vi "FixJKIHelper.vi"() -> ()   [LabVIEW 2017]
uses:
  _Support/Common/Format Timestamp.vi
  _Shared/CSM Shared.lvlib
  _csmDoc/csmdoc.lvlib
  Communicable State Machine.lvlib
  user32.dll
panel:
  out "String Cache":string
  in  "Bottom Right":string
  in  "Bottom Left":string
  out "2D Picture":picture
  in  "Error in":errorcluster caption="error in (no error)"
  out "Listbox":i32(listbox)
  in  "Progress Bar":u8(slide) scale=-1.0..292.0
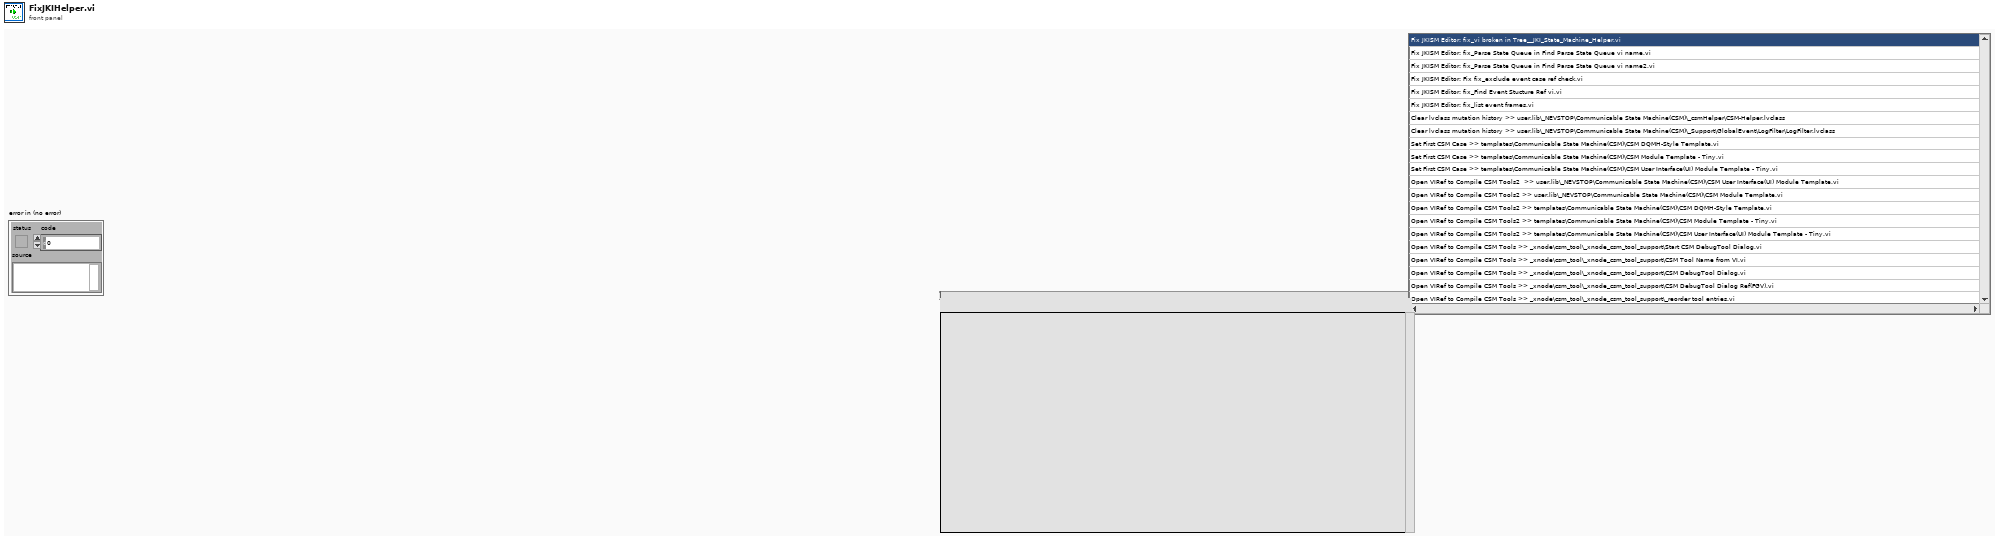
[diagram p1: front panel]
types:
  T1 = enum32{"Invalid", "Standard", "Closed", "Hidden", "Minimized", "Maximized"}
  T2 = enum32{"invalid app kind", "Development System", "Run Time System", "Student Edition", "Embedded LabVIEW", "Evaluation", "Custom"}
  T3 = cluster{"Core":cluster{"Current VI Reference":refnum<vi>, "Close Panel on Exit?":bool}, "Listbox Symbols":i32[], "Listbox Index":i32, "_JKI State Machine Helper VIs":path[], "CSM Templates":path[], "CSM lvclass":path[], "_JKI State Machine Helper Folders":path[], "Actions":string[], "LangID":string, "DescMap":variant, "NoteMap":variant, "Polish":cluster{"Version":refnum<vi>, "Action":refnum<vi>, "Progress Bar":refnum<vi>, "2D Picture":refnum<vi>, "Hold":bool, "Slides":picture[]}}
  T4 = cluster{"Version":refnum<vi>, "Action":refnum<vi>, "Progress Bar":refnum<vi>, "2D Picture":refnum<vi>, "Hold":bool, "Slides":picture[]}
  T5 = cluster{"Current VI Reference":refnum<vi>, "Close Panel on Exit?":bool}
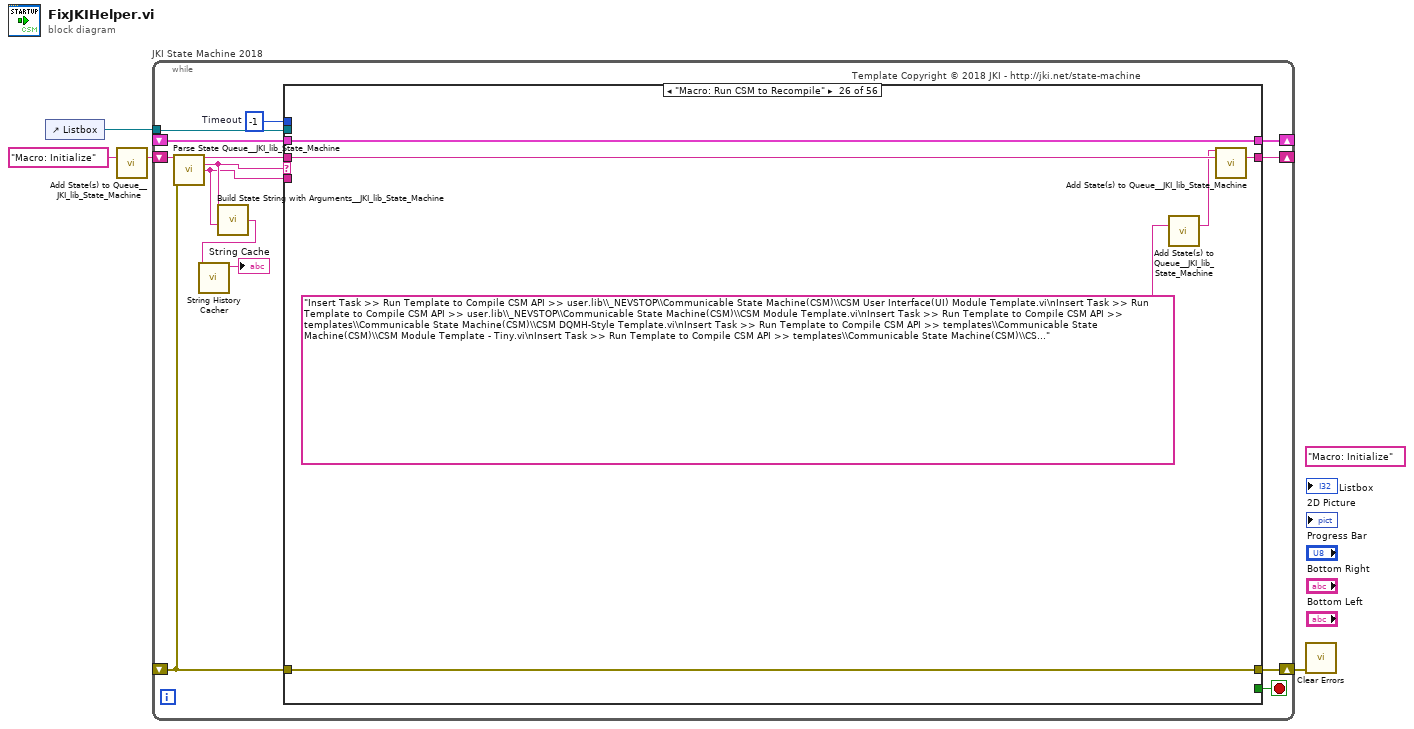
[diagram p0: block diagram]
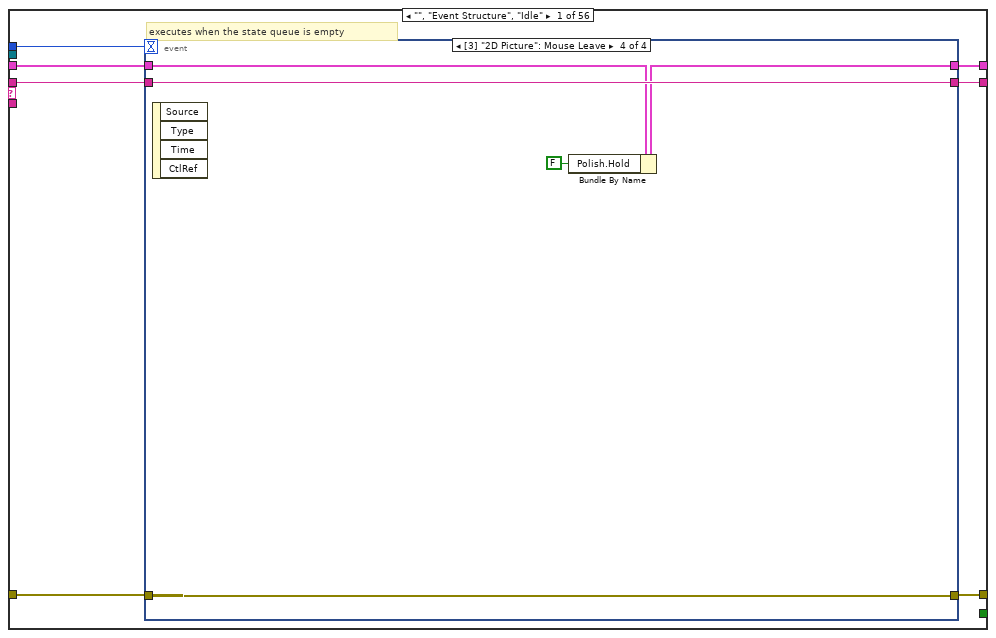
[diagram p2: hidden frame]
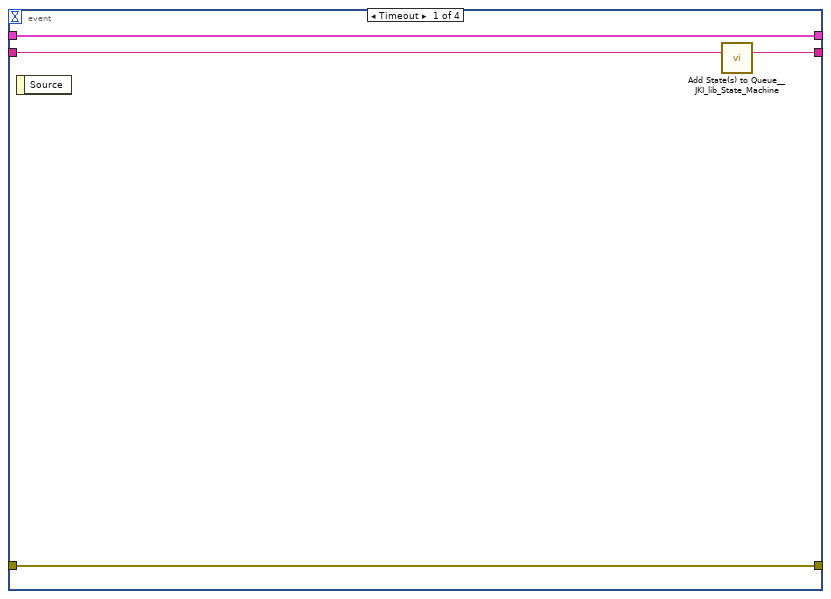
[diagram p3: hidden frame]
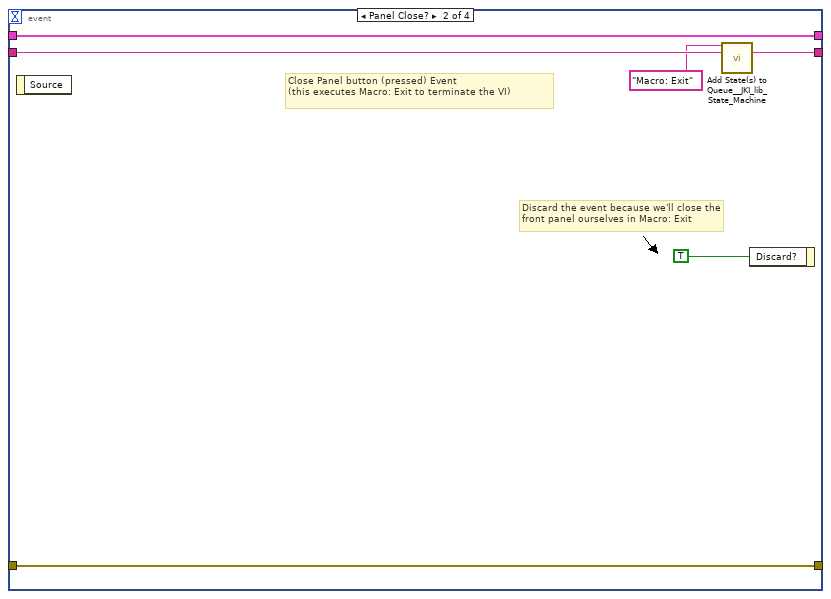
[diagram p4: hidden frame]
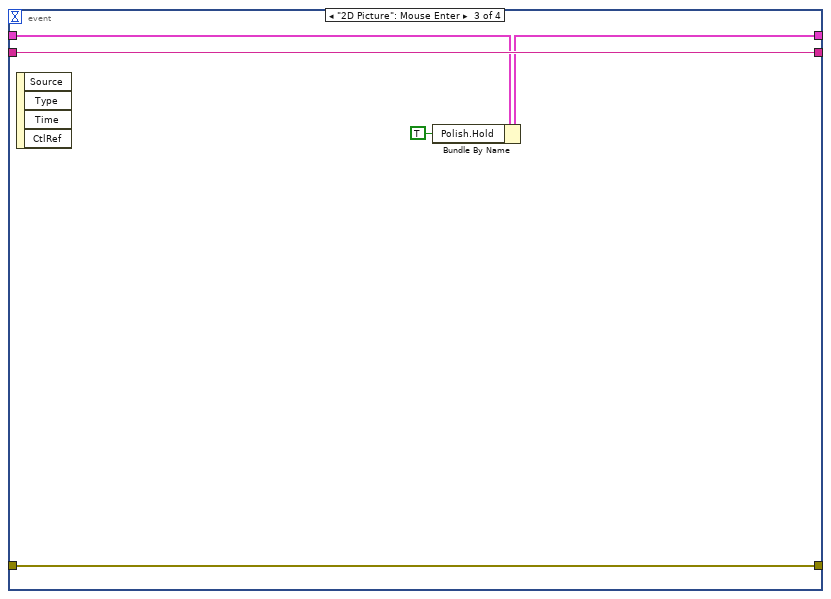
[diagram p5: hidden frame]
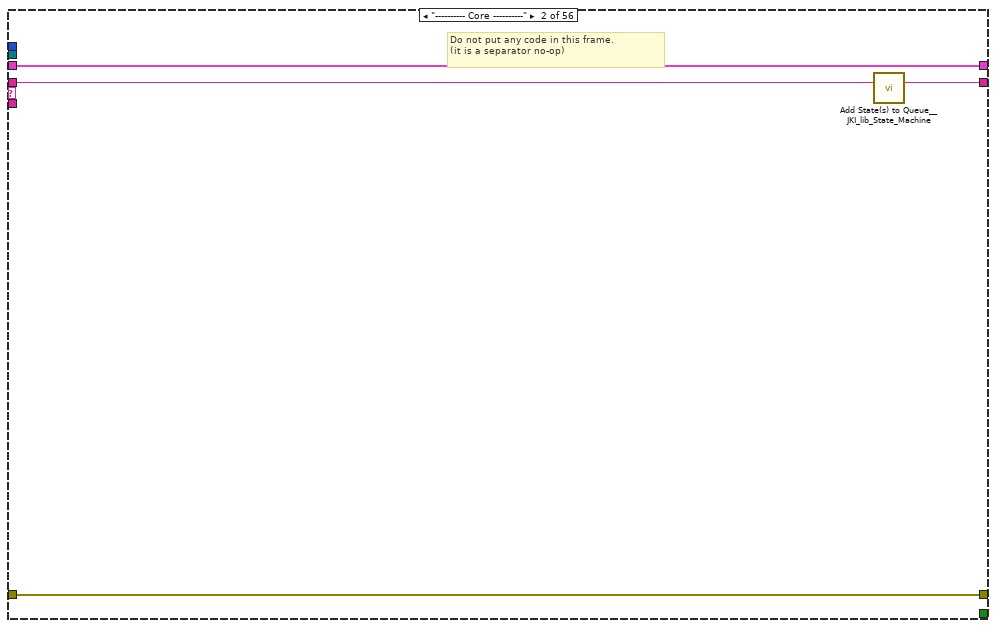
[diagram p6: hidden frame]
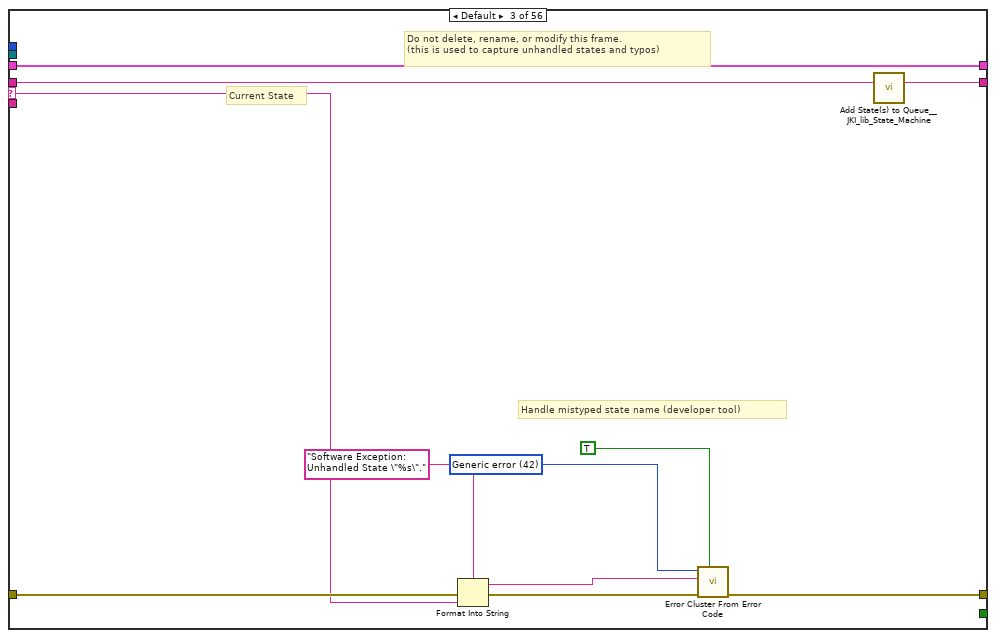
[diagram p7: hidden frame]
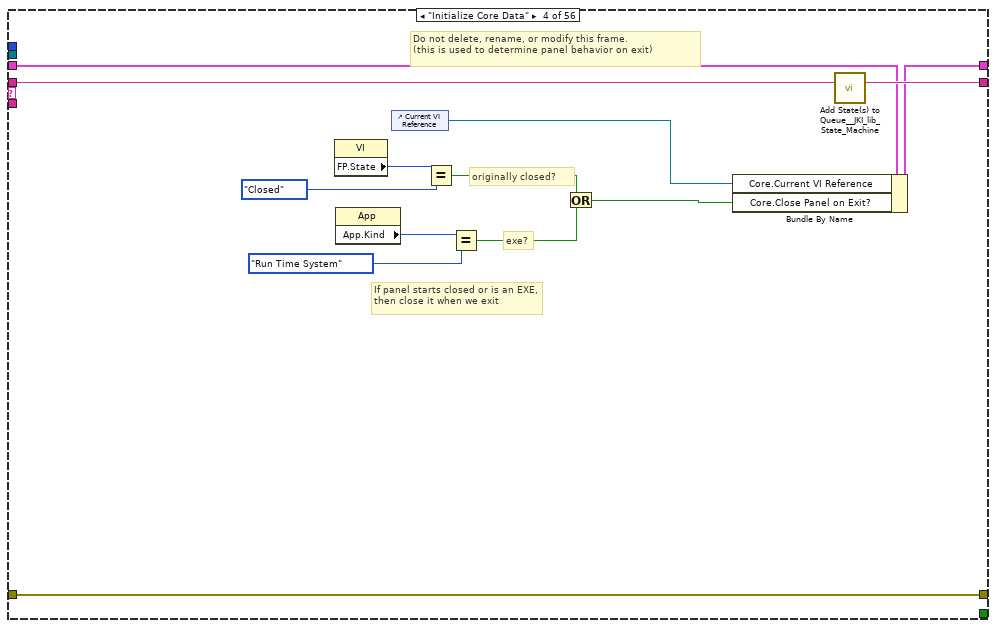
[diagram p8: hidden frame]
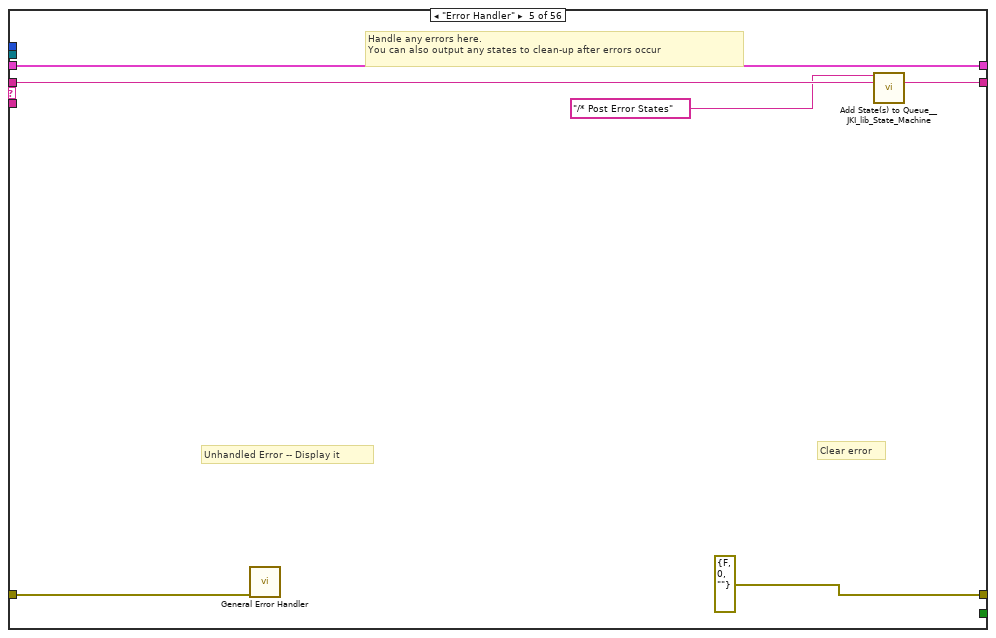
[diagram p9: hidden frame]
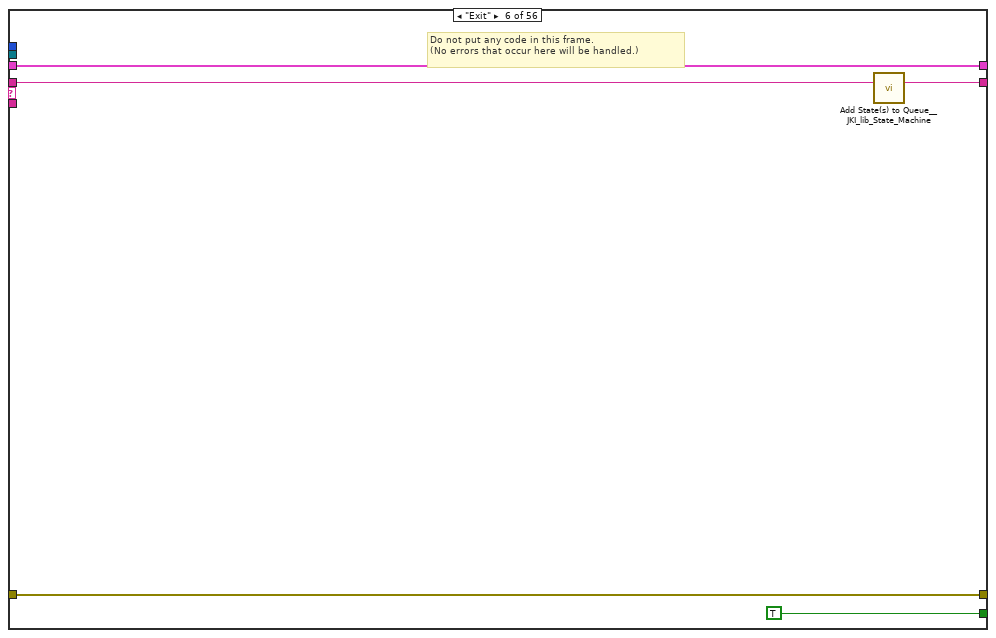
[diagram p10: hidden frame]
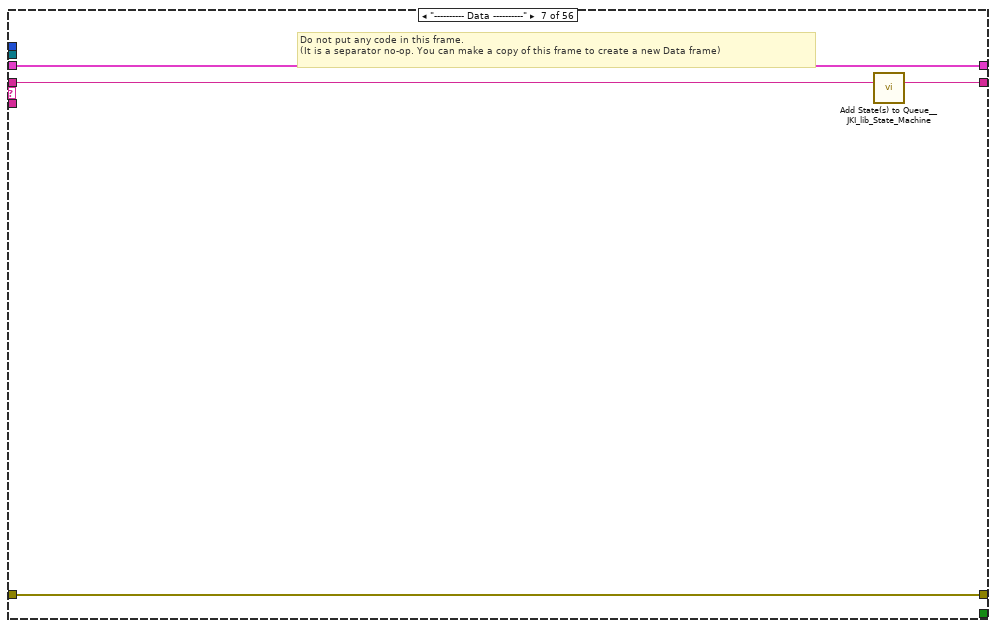
[diagram p11: hidden frame]
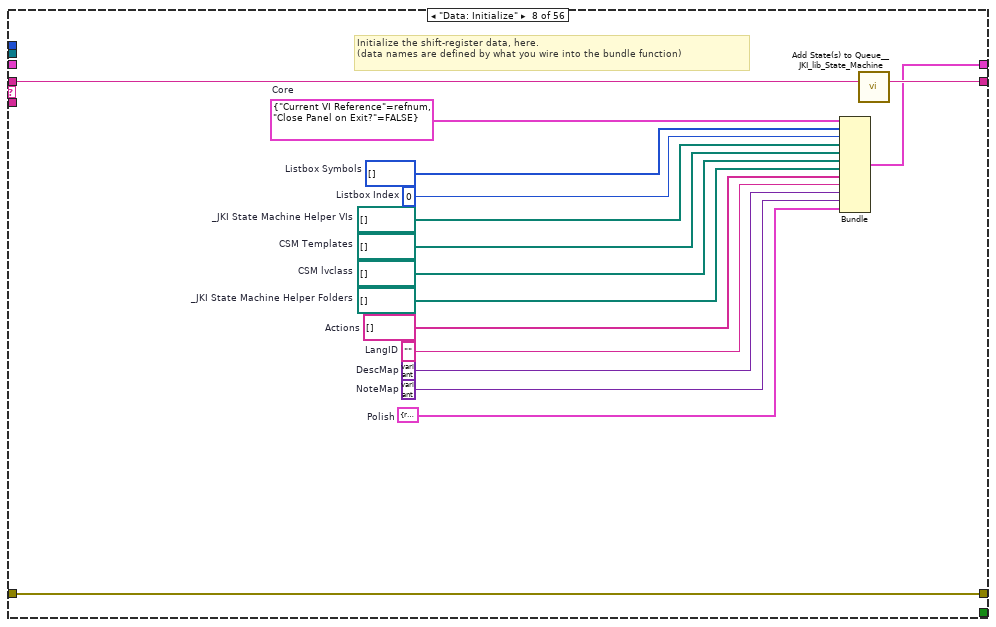
[diagram p12: hidden frame]
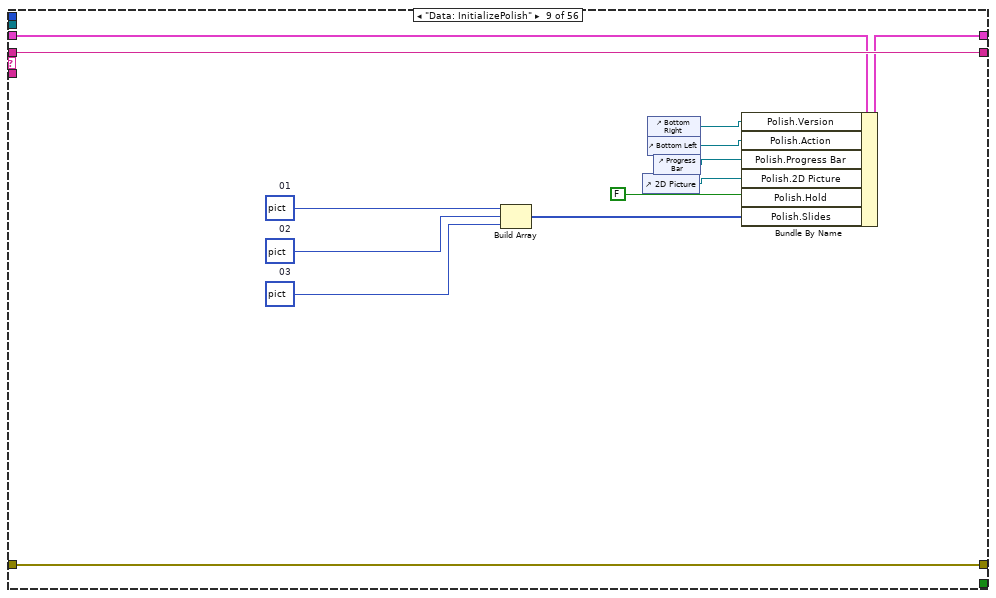
[diagram p13: hidden frame]
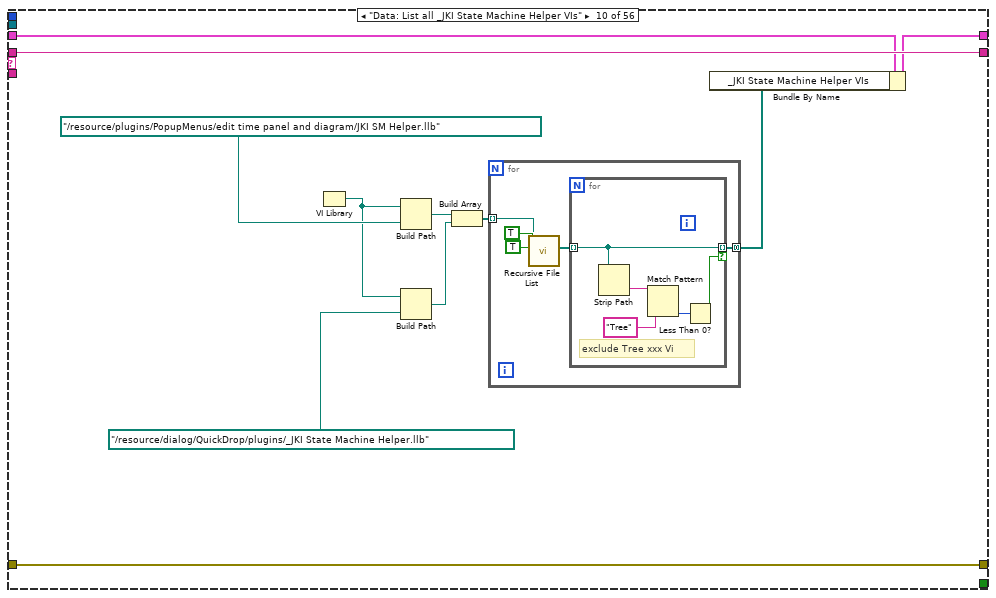
[diagram p14: hidden frame]
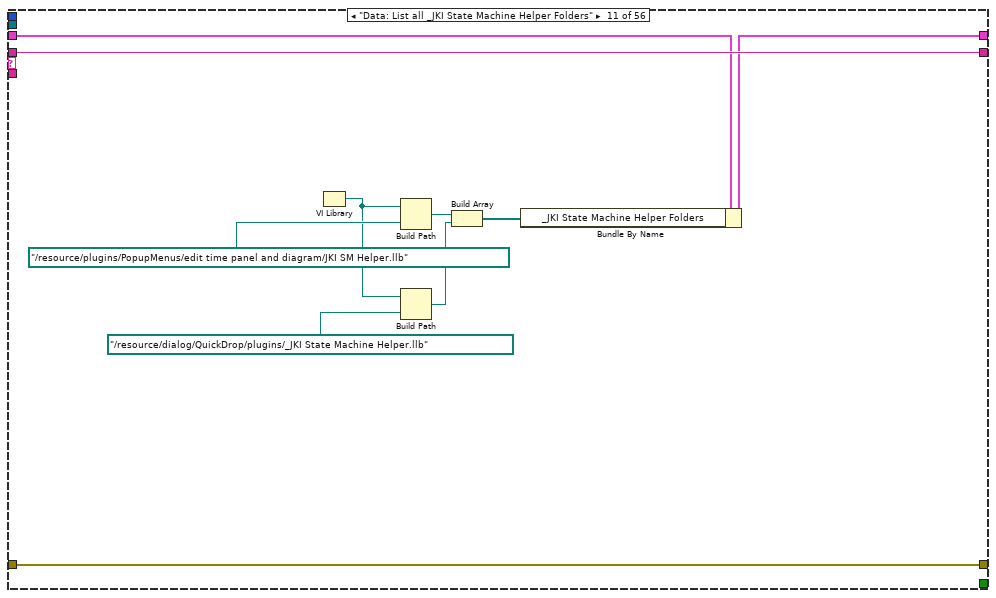
[diagram p15: hidden frame]
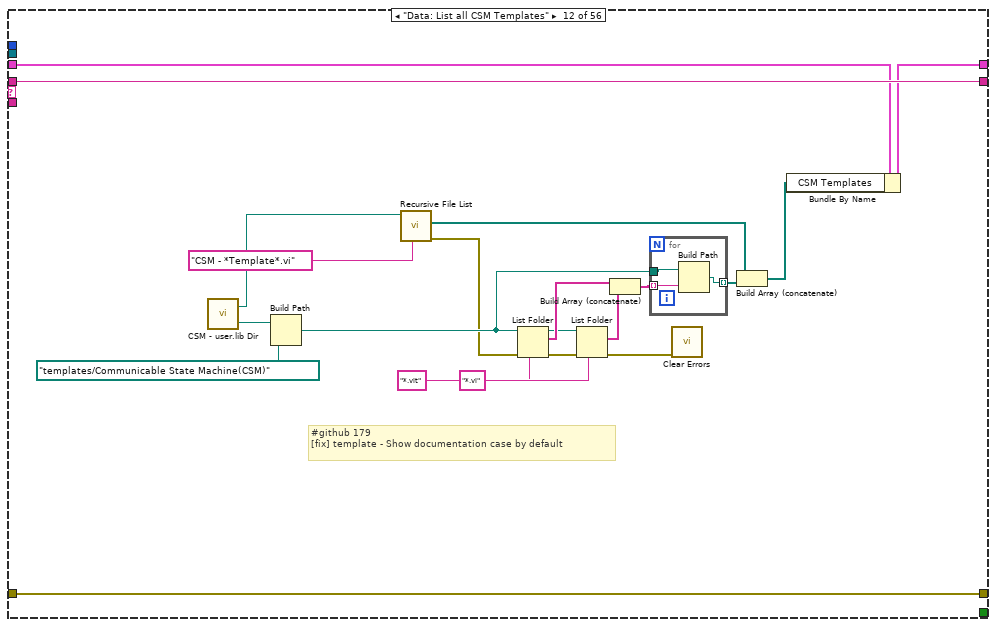
[diagram p16: hidden frame]
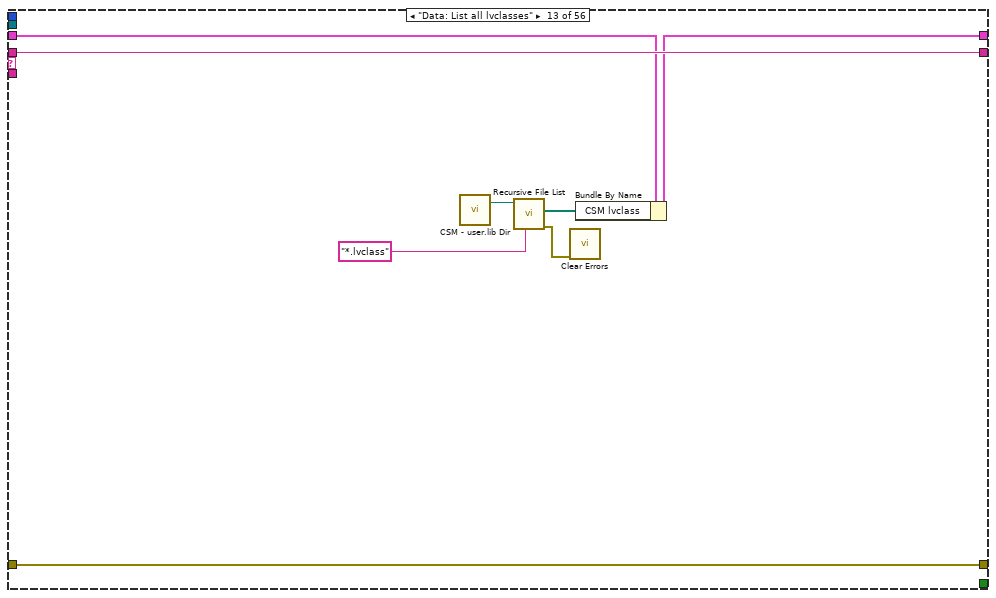
[diagram p17: hidden frame]
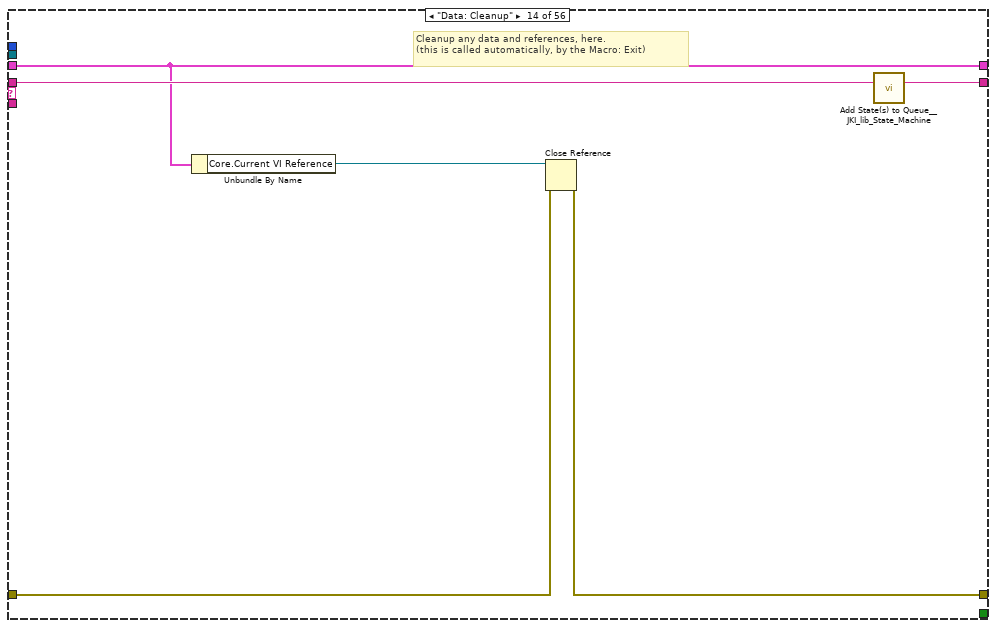
[diagram p18: hidden frame]
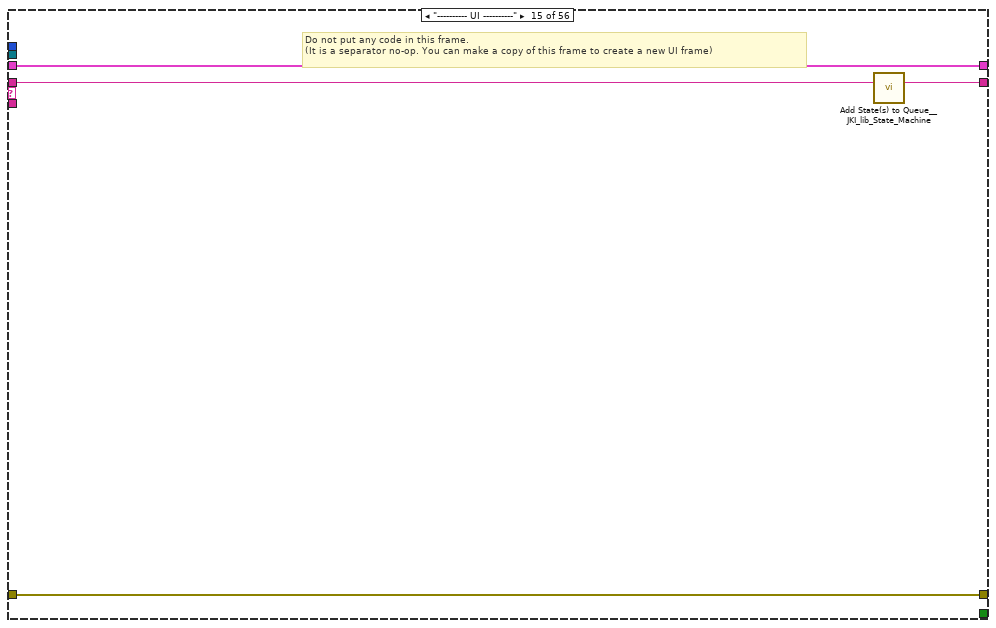
[diagram p19: hidden frame]
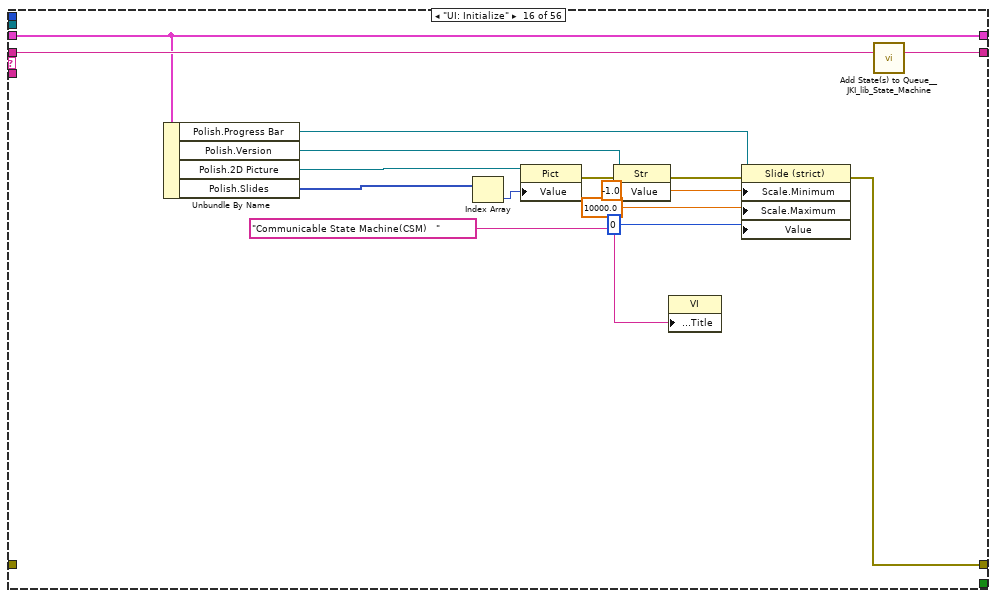
[diagram p20: hidden frame]
diagram:
  (unwired) "Macro: Initialize"
  n1 = control-ref of="Listbox"() -> (w2:refnum<vi>)
  n2 = call <vilib>:"Add State(s) to Queue__JKI_lib_State_Machine.vi"("State(s) in (\"\")"="Macro: Initialize") -> ("States Out"=w4:string)  [unwired: 14 in]
  n3 = while "JKI State Machine 2018" {
    shift-right: [w13] -> _
    shift-left: _ -> [w12]
    shift-right: [w16] -> w1
    shift-left: _ -> [w10]
    shift-right: [w15] -> _
    shift-left: w4 -> [w17]
    tunnel: w2 -> [w9]
    stop <- w14 stop-if-true
    w11 = -1  # Timeout
    # "Template Copyright © 2018 JKI - http://jki.net/state-machine"
    n4 = call <vilib>:"Parse State Queue__JKI_lib_State_Machine.vi"("State Queue"=w17, "Error In (no error)"=w10) -> ("Remaining States"=w18:string, "Current State"=w7:string, "Arguments"=w6:string)  [unwired: 11 in]
    n5 = call <vilib>:"Build State String with Arguments__JKI_lib_State_Machine.vi"("Arguments (\"\")"=w6, "State"=w7) -> ("State with Arguments"=w5:string)  [unwired: 4 in]
    n6 = call "String History Cacher.vi"("String"=w5) -> ("String Cache"=→"String Cache":string)  [unwired: 10 in]
    n7 = case shown="\"Macro: Run CSM to Recompile\"" w7 {
      selector: w7 -> [_ _ w50 _ _ _ _ _ _ _ _ _ _ _ _ _ _ _ _ _ _ _ _ _ _ _ _ _ _ _ _ _ _ _ _ _ _ _ _ _ _ _ _ _ _ _ _ _ _ _ _ _ _ _ _ _]
      tunnel: w18 -> [w25 w49 w54 w73 w79 w84 w88 w104 w116 w128 w148 w168 w179 w186 w190 w205 w215 w222 w229 w263 w330 w370 w375 w377 w391 w414 w420 w426 w437 w439 w450 w462 w471 w486 w500 w513 w527 w540 w542 w562 w572 w577 w582 w587 w592 w597 w602 w607 w616 w629 w658 w677 w690 w707 w715 w723]
      tunnel: w6 -> [_ _ _ _ _ _ _ _ _ _ _ _ _ _ _ _ _ w217 _ w257 _ _ _ _ _ _ _ _ _ _ _ _ _ _ _ w512 _ _ w545 w558 w568 _ _ _ _ _ _ _ w612 w624 w651 w671 _ _ _ w721]
      tunnel: w12 -> [w23 w46 w52 w66 w76 w82 w85 _ w115 w127 w147 w167 w178 w181 w187 w202 w212 w220 w227 w259 w339 w367 w372 w380 w393 w416 w422 w425 w434 w438 w448 w460 w469 w485 w498 w510 w525 w537 w555 w565 w574 w579 w584 w589 w594 w599 w604 w609 w619 w631 w660 w679 w697 w711 w718 w726]
      tunnel: [w22 w47 w56 w70 errorcluster {"status"=FALSE, "code"=0, "source"=""} ("error out") w81 w86 w101 w117 w118 w140 w169 w180 w182 w188 w192 w216 w218 w228 w260 w357 w368 w373 w381 w394 w417 w423 w427 w435 w440 w446 w461 w467 w483 w496 w506 w524 w538 w556 w566 w575 w580 w585 w590 w595 w600 w605 w610 w621 w632 w661 w680 w698 w712 "Error in" w725] -> w16
      tunnel: w10 -> [w21 w47 w55 w70 w75 w81 w86 w101 w117 w118 w140 w169 w180 w183 w188 _ w216 w219 _ w261 w357 w368 w373 w381 w394 w417 w423 w427 w435 w440 w446 w461 w467 w483 w496 w506 w524 w538 w556 w566 w575 w580 w585 w590 w595 w600 w605 w610 w621 w632 w661 w680 w698 w712 _ _]
      tunnel: [w24 w48 w53 w72 w78 w83 w87 w103 w116 w128 w148 w168 w179 w185 w189 w204 w215 w221 w229 w262 w331 w369 w374 w378 w392 w415 w421 w426 w436 w439 w450 w462 w471 w486 w500 w513 w527 w539 w543 w563 w573 w578 w583 w588 w593 w598 w603 w608 w617 w630 w659 w678 w691 w708 w716 w724] -> w15
      tunnel: [_ _ _ _ _ TRUE _ _ _ _ _ _ _ _ _ _ _ _ _ _ _ _ _ _ _ _ _ _ _ _ _ _ _ _ _ _ _ _ _ _ _ _ _ _ _ _ _ _ _ _ _ _ _ _ _ _] -> w14
      tunnel: [w20 w46 w52 w71 w76 w82 w85 w102 w114 w120 w141 w150 w175 w181 w187 w202 w212 w220 w227 w259 w339 w367 w372 w380 w393 w416 w422 w425 w434 w438 w443 w459 w465 w480 w494 w509 w523 w537 w555 w565 w574 w579 w584 w589 w594 w599 w604 w609 w619 w631 w660 w679 w697 w710 w717 w726] -> w13
      tunnel: w11 -> [w19 _ _ _ _ _ _ _ _ _ _ _ _ _ _ _ _ _ _ _ _ _ _ _ _ _ _ _ _ _ _ _ _ _ _ _ _ _ _ _ _ _ _ _ _ _ _ _ _ _ _ _ _ _ _ _]
      tunnel: w9 -> [_ _ _ _ _ _ _ _ _ _ _ _ _ _ _ _ w211 _ _ _ w346 _ _ _ _ _ _ _ _ _ _ _ _ _ _ _ _ _ _ _ _ _ _ _ _ _ _ _ _ _ _ _ _ _ _ _]
      frame "", "Event Structure", "Idle" {
        # "executes when the state queue is empty"
        n8 = event shown="[3] \"2D Picture\": Mouse Leave" {
          selector: _ -> [_ _ _ _]
          dyn-events: _ -> [_ _ _ _]
          timeout: w19 -> [_ _ _ _]
          tunnel: w25 -> [w29 w35 w40 w45]
          tunnel: [w28 w34 w40 w45] -> w24
          tunnel: w23 -> [w26 w32 w38 w43]
          tunnel: [w27 w33 w39 w44] -> w22
          tunnel: w21 -> [w27 w33 w39 w44]
          tunnel: [w26 w32 w36 w41] -> w20
          event Timeout {
            n9 = event-data() -> ()  [unwired: 1 in, 1 out]
            n10 = call <vilib>:"Add State(s) to Queue__JKI_lib_State_Machine.vi"("State(s) in (\"\")"=w29) -> ("States Out"=w28:string)  [unwired: 14 in]
          }
          event Panel Close? {
            # "Discard the event because we'll close the front panel ourselves in Macro: Exit"
            # "Close Panel button (pressed) Event\n(this executes Macro: Exit to terminate the VI)"
            n11 = event-data() -> ()  [unwired: 1 in, 1 out]
            n12 = call <vilib>:"Add State(s) to Queue__JKI_lib_State_Machine.vi"("State(s) in Front (\"\")"="Macro: Exit", "State(s) in (\"\")"=w35) -> ("States Out"=w34:string)  [unwired: 13 in]
            n13 = event-data("Discard?"=TRUE) -> ()  [unwired: 1 in, 1 out]
          }
          event "2D Picture": Mouse Enter {
            n14 = event-data() -> ()  [unwired: 1 in, 4 out]
            n15 = Bundle By Name(cluster=w38, "Polish.Hold"=TRUE) -> (w36:T3)
          }
          event "2D Picture": Mouse Leave {
            n16 = event-data() -> ()  [unwired: 1 in, 4 out]
            n17 = Bundle By Name(cluster=w43, "Polish.Hold"=FALSE) -> (w41:T3)
          }
        }
      }
      frame "---------- Core ----------" {
        # "Do not put any code in this frame.\n(it is a separator no-op)"
        n18 = call <vilib>:"Add State(s) to Queue__JKI_lib_State_Machine.vi"("State(s) in (\"\")"=w49) -> ("States Out"=w48:string)  [unwired: 14 in]
      }
      frame Default {
        w59 = 42 items=["No error", "Argument error", "Memory is full", "Out of zone", "End of file", "File already open", "Generic file I/O error", "File not found", "File permission error", "Disk is full", "Duplicate path", "Too many files open", "System feature not enabled", "Resource file not found", "Cannot add resource", "Resource not found", "Image not found", "Image memory error", "Pen does not exist", "Config type invalid", "Config token not found", "Config parse error", "Config memory error", "Bad external code format", "Bad external code offset", "External code not present", "Null window", "Destroy window error", "Null menu", "Print aborted", "Bad print record", "Print driver error", "Windows error during printing", "Memory error during printing", "Print dialog error", "Generic print error", "Invalid device refnum", "Device not found", "Device parameter error", "Device unit error", "Cannot open device", "Device call aborted", "Generic error", "Cancelled by user", "Object ID too low", "Object ID too high", "Object not in heap", "Unknown heap", "Unknown object (invalid DefProc)", "Unknown object (DefProc not in table)", "Message out of range", "Invalid (null) method", "Unknown message", "Manager call not supported", "Bad address", "Network operation in progress", "Network operation timed out", "Connection is busy", "Network attribute not supported", "Network error", "Address in use", "System out of memory", "Connection aborted", "Connection refused", "Not connected", "Already connected", "Connection closed", "Initialization error (interapplication manager)", "Bad occurrence", "Wait on unbound occurrence handler", "Occurrence queue overflow", "Datalog type conflict", "Unused", "Unrecognized type (interapplication manager)", "Memory corrupt", "Failed to make temporary DLL", "Old CIN version", "Drag socket not found", "Failed to load drop-object", "Failed to register OLE object", "Failed to release OLE object", "Format specifier type mismatch", "Unknown format specifier", "Too few format specifiers", "Too many format specifiers", "Scan failed", "Newer CIN version", "Error converting to variant", "Runtime menu error", "Password tampered", "Variant attribute not found", "Incompatible variant data type", "Event data is not available", "Event Store is not present", "Occurrence is not found", "Event Queue is not created", "Event info is not available", "Refnum passed is NULL", "Error retrieving Class GUID", "Error retrieving CoClass GUID", "Error retrieving TypeLib GUID.", "Bad built application magic bytes.", "Specific driver is different from the specific driver associated with the Logical Name.", "There is no session opened to the class driver.", "Max Error", "MAX - Error with config objects", "MAX - Error loading configuration", "MAX - Group not supported"]
        # "Current State"
        # "Do not delete, rename, or modify this frame.\n(this is used to capture unhandled states and typos)"
        # "Handle mistyped state name (developer tool)"
        n19 = Format Into String(format string="Software Exception: Unhandled State \"%s\"." ("message"), error in=w55, w50) -> (resulting string=w58:string, error out=w57:errorcluster)  [unwired: 1 in]
        n20 = call <vilib>:"Error Cluster From Error Code.vi"("show call chain? (False)"=TRUE, "error in (no error)"=w57, "error message (\"\")"=w58, "error code (0)"=w59) -> ("error out"=w56:errorcluster)  [unwired: 5 in]
        n21 = call <vilib>:"Add State(s) to Queue__JKI_lib_State_Machine.vi"("State(s) in (\"\")"=w54) -> ("States Out"=w53:string)  [unwired: 14 in]
      }
      frame "Initialize Core Data" {
        # "Do not delete, rename, or modify this frame.\n(this is used to determine panel behavior on exit)"
        # "originally closed?"
        # "exe?"
        # "If panel starts closed or is an EXE, then close it when we exit"
        n22 = property class="VI"() -> ("FP.State"=w63:T1)  [unwired: 2 in, 2 out]
        n23 = property class="App"() -> ("App.Kind"=w69:T2)  [unwired: 2 in, 2 out]
        n24 = control-ref of="Current VI Reference"() -> (w64:refnum<vi>)
        n25 = Equal?(x=w63, y=T1."Closed" ("Front Panel Window:State")) -> (x = y?=w61:bool)
        n26 = Equal?(x=w69, y=T2."Run Time System" ("Application:Kind")) -> (x = y?=w67:bool)
        n27 = Or(x=w61, y=w67) -> (x .or. y?=w65:bool)
        n28 = Bundle By Name(cluster=w66, "Core.Current VI Reference"=w64, "Core.Close Panel on Exit?"=w65) -> (w71:T3)
        n29 = call <vilib>:"Add State(s) to Queue__JKI_lib_State_Machine.vi"("State(s) in (\"\")"=w73) -> ("States Out"=w72:string)  [unwired: 14 in]
      }
      frame "Error Handler" {
        # "Unhandled Error -- Display it"
        # "Handle any errors here.\nYou can also output any states to clean-up after errors occur"
        # "Clear error"
        n30 = call <vilib>:"General Error Handler.vi"("error in (no error)"=w75) -> ()  [unwired: 10 in, 5 out]
        n31 = call <vilib>:"Add State(s) to Queue__JKI_lib_State_Machine.vi"("State(s) in Front (\"\")"="/* Post Error States", "State(s) in (\"\")"=w79) -> ("States Out"=w78:string)  [unwired: 13 in]
      }
      frame "Exit" {
        # "Do not put any code in this frame.\n(No errors that occur here will be handled.)"
        n32 = call <vilib>:"Add State(s) to Queue__JKI_lib_State_Machine.vi"("State(s) in (\"\")"=w84) -> ("States Out"=w83:string)  [unwired: 14 in]
      }
      frame "---------- Data ----------" {
        # "Do not put any code in this frame.\n(It is a separator no-op. You can make a copy of this frame to create a new Data frame)"
        n33 = call <vilib>:"Add State(s) to Queue__JKI_lib_State_Machine.vi"("State(s) in (\"\")"=w88) -> ("States Out"=w87:string)  [unwired: 14 in]
      }
      frame "Data: Initialize" {
        w89 = T4 {"Version"=refnum, "Action"=refnum, "Progress Bar"=refnum, "2D Picture"=refnum, "Hold"=TRUE, "Slides"=[]}  # Polish
        w90 = variant  # NoteMap
        w91 = variant  # DescMap
        w92 = ""  # LangID
        w93 = string[] []  # Actions
        w94 = path[] []  # _JKI State Machine Helper Folders
        w95 = path[] []  # CSM lvclass
        w96 = i32[] []  # Listbox Symbols
        w97 = 0  # Listbox Index
        w98 = path[] []  # CSM Templates
        w99 = path[] []  # _JKI State Machine Helper VIs
        w100 = T5 {"Current VI Reference"=refnum, "Close Panel on Exit?"=FALSE}  # Core
        # "Initialize the shift-register data, here.\n(data names are defined by what you wire into the bundle function)"
        n34 = Bundle("Core"=w100, "Listbox Symbols"=w96, "Listbox Index"=w97, "_JKI State Machine Helper VIs"=w99, "CSM Templates"=w98, "CSM lvclass"=w95, "_JKI State Machine Helper Folders"=w94, "Actions"=w93, "LangID"=w92, "DescMap"=w91, "NoteMap"=w90, "Polish"=w89) -> (w102:T3)  [unwired: 1 in]
        n35 = call <vilib>:"Add State(s) to Queue__JKI_lib_State_Machine.vi"("State(s) in (\"\")"=w104) -> ("States Out"=w103:string)  [unwired: 14 in]
      }
      frame "Data: InitializePolish" {
        w105 = picture bytes[1036830]  # 03
        w106 = picture bytes[1036830]  # 02
        w107 = picture bytes[1036830]  # 01
        n36 = Build Array(w107, w106, w105) -> (w110:picture[])
        n37 = control-ref of="2D Picture"() -> (w112:refnum<vi>)
        n38 = control-ref of="Bottom Right"() -> (w109:refnum<vi>)
        n39 = control-ref of="Bottom Left"() -> (w108:refnum<vi>)
        n40 = control-ref of="Progress Bar"() -> (w113:refnum<vi>)
        n41 = Bundle By Name(cluster=w115, "Polish.Version"=w109, "Polish.Action"=w108, "Polish.Progress Bar"=w113, "Polish.2D Picture"=w112, "Polish.Hold"=FALSE, "Polish.Slides"=w110) -> (w114:T3)
      }
      frame "Data: List all _JKI State Machine Helper VIs" {
        n42 = VI Library() -> (path=w125:path)
        n43 = Build Path(base path=w125, name or relative path=path "../resource/plugins/PopupMenus/edit time panel and diagram/JKI SM Helper.llb") -> (appended path=w123:path)
        n44 = Build Path(base path=w125, name or relative path=path "../resource/dialog/QuickDrop/plugins/_JKI State Machine Helper.llb") -> (appended path=w121:path)
        n45 = Build Array(w123, w121) -> (w122:path[])
        n46 = for {
          tunnel: w122 -> [w131] mode=indexing
          tunnel: [w129] -> w119 mode=concatenating
          n47 = call <vilib>:"Recursive File List.vi"("Continue Recursing on Error? (F)"=TRUE, "Treat LLBs as Folders?"=TRUE, "Folder Path"=w131) -> ("All Files in Dir"=w130:path[])  [unwired: 4 in, 4 out]
          n48 = for {
            tunnel: w130 -> [w135] mode=indexing
            tunnel: [w135] -> w129 mode=indexing if=w134
            # "exclude Tree xxx Vi"
            n49 = Strip Path(path=w135) -> (name=w138:string)  [unwired: 1 out]
            n50 = Match Pattern(string=w138, regular expression="Tree") -> (offset past match=w136:i32)  [unwired: 1 in, 3 out]
            n51 = Less Than 0?(x=w136) -> (x < 0?=w134:bool)
          }
        }
        n52 = Bundle By Name(cluster=w127, "_JKI State Machine Helper VIs"=w119) -> (w120:T3)
      }
      frame "Data: List all _JKI State Machine Helper Folders" {
        n53 = VI Library() -> (path=w145:path)
        n54 = Build Path(base path=w145, name or relative path=path "../resource/plugins/PopupMenus/edit time panel and diagram/JKI SM Helper.llb") -> (appended path=w143:path)
        n55 = Build Path(base path=w145, name or relative path=path "../resource/dialog/QuickDrop/plugins/_JKI State Machine Helper.llb") -> (appended path=w142:path)
        n56 = Build Array(w143, w142) -> (w139:path[])
        n57 = Bundle By Name(cluster=w147, "_JKI State Machine Helper Folders"=w139) -> (w141:T3)
      }
      frame "Data: List all CSM Templates" {
        # "#github 179\n[fix] template - Show documentation case by default"
        n58 = call "CSM - user.lib Dir.vi"() -> ("<LabVIEW>"=w157:path, "csm_user.lib_dir"=w159:path)  [unwired: 2 in]
        n59 = Build Path(base path=w157, name or relative path=path "templates/Communicable State Machine(CSM)") -> (appended path=w166:path)
        n60 = call <vilib>:"Recursive File List.vi"("pattern"="CSM - *Template*.vi" ("name or relative path"), "Folder Path"=w159) -> ("error out"=w160:errorcluster, "All Files in Dir"=w161:path[])  [unwired: 5 in, 3 out]
        n61 = List Folder(path=w166, pattern="*.vit", error in=w160) -> (path out=w153:path, filenames=w162:string[], error out=w155:errorcluster)  [unwired: 1 in, 1 out]
        n62 = List Folder(path=w153, pattern="*.vi", error in=w155) -> (filenames=w163:string[], error out=w156:errorcluster)  [unwired: 1 in, 2 out]
        n63 = Build Array (concatenate)(w162, w163) -> (w164:string[])
        n64 = for {
          tunnel: w164 -> [w172] mode=indexing
          tunnel: [w171] -> w165 mode=indexing
          tunnel: w166 -> [w170]
          n65 = Build Path(base path=w170, name or relative path=w172) -> (appended path=w171:path)
        }
        n66 = call <vilib>:"Clear Errors.vi"("error in (no error)"=w156) -> ()  [unwired: 5 in, 2 out]
        n67 = Build Array (concatenate)(w161, w165) -> (w149:path[])
        n68 = Bundle By Name(cluster=w167, "CSM Templates"=w149) -> (w150:T3)
      }
      frame "Data: List all lvclasses" {
        n69 = call "CSM - user.lib Dir.vi"() -> ("csm_user.lib_dir"=w177:path)  [unwired: 2 in, 1 out]
        n70 = call <vilib>:"Recursive File List.vi"("pattern"="*.lvclass", "Folder Path"=w177) -> ("error out"=w173:errorcluster, "All Files in Dir"=w174:path[])  [unwired: 5 in, 3 out]
        n71 = call <vilib>:"Clear Errors.vi"("error in (no error)"=w173) -> ()  [unwired: 5 in, 2 out]
        n72 = Bundle By Name(cluster=w178, "CSM lvclass"=w174) -> (w175:T3)
      }
      frame "Data: Cleanup" {
        # "Cleanup any data and references, here.\n(this is called automatically, by the Macro: Exit)"
        n73 = Unbundle By Name(w181) -> ("Core.Current VI Reference"=w184:refnum<vi>)
        n74 = Close Reference(reference=w184, error in (no error)=w183) -> (error out=w182:errorcluster)
        n75 = call <vilib>:"Add State(s) to Queue__JKI_lib_State_Machine.vi"("State(s) in (\"\")"=w186) -> ("States Out"=w185:string)  [unwired: 14 in]
      }
      frame "---------- UI ----------" {
        # "Do not put any code in this frame.\n(It is a separator no-op. You can make a copy of this frame to create a new UI frame)"
        n76 = call <vilib>:"Add State(s) to Queue__JKI_lib_State_Machine.vi"("State(s) in (\"\")"=w190) -> ("States Out"=w189:string)  [unwired: 14 in]
      }
      frame "UI: Initialize" {
        w191 = "Communicable State Machine(CSM)   " ("Value")
        n77 = Unbundle By Name(w202) -> ("Polish.Progress Bar"=w196:refnum<vi>, "Polish.Version"=w199:refnum<vi>, "Polish.2D Picture"=w201:refnum<vi>, "Polish.Slides"=w203:picture[])
        n78 = Index Array(array=w203) -> (element=w200:picture)  [unwired: 1 in]
        n79 = property class="Pict"(reference=w201, "Value"=w200) -> (error out=w198:errorcluster)  [unwired: 1 in, 1 out]
        n80 = property class="Str"(reference=w199, error in=w198, "Value"=w191) -> (error out=w197:errorcluster)  [unwired: 1 out]
        n81 = property class="VI"("Front Panel.Title"=w191) -> ()  [unwired: 2 in, 2 out]
        n82 = property class="Slide (strict)"(reference=w196, error in=w197, "Scale.Minimum"=-1.0 ("Scale.Range:Minimum"), "Scale.Maximum"=10000.0 ("Scale.Range:Maximum"), "Value"=u8 0) -> (error out=w192:errorcluster)  [unwired: 1 out]
        n83 = call <vilib>:"Add State(s) to Queue__JKI_lib_State_Machine.vi"("State(s) in (\"\")"=w205) -> ("States Out"=w204:string)  [unwired: 14 in]
      }
      frame "UI: Refresh Listbox" {
        w210 = 0 ("Top Row")
        n84 = Unbundle By Name(w212) -> ("Actions"=w208:string[], "Polish.Progress Bar"=w206:refnum<vi>)
        n85 = Array Size(array=w208) -> (size(s)=w207:i32)
        n86 = Initialize Array(0 ("Top Row"), w207) -> (w213:i32[])
        n87 = To Double Precision Float(number=w207) -> (double precision float=w209:dbl)
        n88 = property on="Property Node" class="LstBox (strict)"(reference=w211, "Item Names"=w208, "Top Row"=w210, "Item Symbols"=w213, "Value"=w210) -> ()  [unwired: 1 in, 2 out]
        n89 = property class="Slide (strict)"(reference=w206, "Scale.Maximum"=w209) -> ()  [unwired: 1 in, 2 out]
      }
      frame "UI: Cursor Set" {
        # "Argument"
        # "Set and Unset Cursor Busy.\n(Usage: \"UI: Cursor Set >> Busy|Idle\")"
        n90 = case shown="\"Idle\", Default" w217 {
          tunnel: w219 -> [w224 w226]
          tunnel: [w223 w225] -> w218
          frame "Idle", Default {
            n91 = call <vilib>:"Unset Busy.vi"("error in (no error)"=w224) -> ("error out"=w223:errorcluster)  [unwired: 10 in]
          }
          frame "Busy" {
            n92 = call <vilib>:"Set Busy.vi"("error in (no error)"=w226) -> ("error out"=w225:errorcluster)  [unwired: 9 in, 1 out]
          }
        }
        n93 = call <vilib>:"Add State(s) to Queue__JKI_lib_State_Machine.vi"("State(s) in (\"\")"=w222) -> ("States Out"=w221:string)  [unwired: 14 in]
      }
      frame "UI: Bring Window to Topmost(Windows Only)" {
        n94 = disable-structure shown="OS==Win" {
          disable-tunnel: [w235 _] -> w228
          disable-tunnel: w227 -> [w234 _]
          frame condition #0 (active) {
            w240 = 0 items=["NULL"]
            # "How to Bring the Front Panel in Front of All Desktop Windows? -Batch File Method\nhttps://knowledge.ni.com/KnowledgeArticleDetails?id=kA03q000000YOu6CAG&l=en-US"
            n95 = Unbundle By Name(w234) -> ("Core.Current VI Reference"=w233:refnum<vi>)
            n96 = property class="VI"(reference=w233) -> (error out=w236:errorcluster, "Front Panel.Title"=w237:string)  [unwired: 1 in, 1 out]
            n97 = call "CSM - user.lib Dir.vi"() -> ("csm_user.lib_dir"=w232:path)  [unwired: 2 in, 1 out]
            n98 = dll-call lib="user32.dll" fn="FindWindowA" label="FindWindow"(error in=w236, "lpszClassName"=w240, "lpszWindowName"=w237) -> (error out=w239:errorcluster, "hWnd"=w238:u64)  [unwired: 3 in, 2 out]
            n99 = Build Path(base path=w232, name or relative path=path "_scripts/sendkeys.bat") -> (appended path=w230:path)
            n100 = case shown="Default" w238 {
              selector: w238 -> [_ w247]
              tunnel: w239 -> [w241 w248]
              tunnel: [w241 w246] -> w235
              tunnel: w230 -> [_ w244]
              frame 0 {
              }
              frame Default {
                n101 = dll-call lib="user32.dll" fn="SetForegroundWindow"(error in=w248, "Handle"=w247) -> (error out=w245:errorcluster)  [unwired: 3 in, 2 out]
                n102 = call <vilib>:"Check if File or Folder Exists.vi"("path"=w244) -> ("file or folder exists?"=w242:bool, "dup path"=w243:path)  [unwired: 8 in, 1 out]
                n103 = case shown="True" w242 {
                  tunnel: [w249 w254] -> w246
                  tunnel: w245 -> [w249 w253]
                  tunnel: w243 -> [_ w250]
                  frame False {
                  }
                  frame True {
                    n104 = Format Into String(format string="\"%s\" \"LabVIEW\" \"\"" ("command line"), w250) -> (resulting string=w251:string)  [unwired: 2 in, 1 out]
                    n105 = call <vilib>:"System Exec.vi"("run minimized? (F)"=TRUE, "wait until completion? (T)"=TRUE, "error in (no error)"=w253, "command line"=w251) -> ("error out"=w254:errorcluster)  [unwired: 4 in, 3 out]
                  }
                }
              }
            }
          }
          frame condition #1 {
          }
        }
      }
      frame "UI: Front Panel State" {
        # "Argument"
        # "Set Front Panel Open or Closed\n(Usage: \"UI: Front Panel State >> Open|Close\")"
        n106 = Unbundle By Name(w259) -> ("Core.Current VI Reference"=w258:refnum<vi>)
        n107 = case shown="\"Minimize\", \"Minimized\"" w257 {
          tunnel: w261 -> [w269 w284 w295 w308 w321]
          tunnel: [w271 w285 w297 w310 w323] -> w260
          tunnel: w258 -> [w270 w282 w296 w309 w322]
          frame "Open", "Standard", Default {
            w264 = T1."Standard" ("State")
            n108 = property class="VI"(reference=w270, error in=w269) -> (reference out=w267:refnum<vi>, error out=w268:errorcluster, "FP.State"=w266:T1)
            n109 = Not Equal?(x=w266, y=w264) -> (x != y?=w265:bool)
            n110 = case shown="True" w265 {
              tunnel: [w275 w277] -> w271
              tunnel: w268 -> [w274 w277]
              tunnel: w267 -> [w273 _]
              tunnel: w264 -> [w272 _]
              frame True {
                n111 = invoke class="VI" method="FP.Open"(reference=w273, error in=w274, "Activate"=TRUE, "State"=w272) -> (error out=w275:errorcluster)  [unwired: 1 in, 4 out]
              }
              frame False {
              }
            }
          }
          frame "Close", "Closed" {
            n112 = property class="VI"(reference=w282, error in=w284) -> (reference out=w281:refnum<vi>, error out=w283:errorcluster, "FP.State"=w279:T1)
            n113 = Not Equal?(x=w279, y=T1."Closed" ("Front Panel Window:State")) -> (x != y?=w278:bool)
            n114 = case shown="True" w278 {
              tunnel: [w286 w289] -> w285
              tunnel: w283 -> [w286 w288]
              tunnel: w281 -> [_ w287]
              frame False {
              }
              frame True {
                n115 = invoke class="VI" method="FP.Close"(reference=w287, error in=w288) -> (error out=w289:errorcluster)  [unwired: 1 in, 2 out]
              }
            }
          }
          frame "Hidden", "Hide" {
            w290 = T1."Hidden" ("State")
            n116 = property class="VI"(reference=w296, error in=w295) -> (reference out=w293:refnum<vi>, error out=w294:errorcluster, "FP.State"=w292:T1)
            n117 = Not Equal?(x=w292, y=w290) -> (x != y?=w291:bool)
            n118 = case shown="True" w291 {
              tunnel: [w301 w302] -> w297
              tunnel: w294 -> [w300 w302]
              tunnel: w293 -> [w299 _]
              tunnel: w290 -> [w298 _]
              frame True {
                n119 = invoke class="VI" method="FP.Open"(reference=w299, error in=w300, "State"=w298) -> (error out=w301:errorcluster)  [unwired: 2 in, 4 out]
              }
              frame False {
              }
            }
          }
          frame "Minimize", "Minimized" {
            w303 = T1."Minimized" ("State")
            n120 = property class="VI"(reference=w309, error in=w308) -> (reference out=w306:refnum<vi>, error out=w307:errorcluster, "FP.State"=w305:T1)
            n121 = Not Equal?(x=w305, y=w303) -> (x != y?=w304:bool)
            n122 = case shown="True" w304 {
              tunnel: [w314 w315] -> w310
              tunnel: w307 -> [w313 w315]
              tunnel: w306 -> [w312 _]
              tunnel: w303 -> [w311 _]
              frame True {
                n123 = invoke class="VI" method="FP.Open"(reference=w312, error in=w313, "State"=w311) -> (error out=w314:errorcluster)  [unwired: 2 in, 4 out]
              }
              frame False {
              }
            }
          }
          frame "Maximize", "Maximized" {
            w316 = T1."Maximized" ("State")
            n124 = property class="VI"(reference=w322, error in=w321) -> (reference out=w319:refnum<vi>, error out=w320:errorcluster, "FP.State"=w318:T1)
            n125 = Not Equal?(x=w318, y=w316) -> (x != y?=w317:bool)
            n126 = case shown="True" w317 {
              tunnel: [w327 w328] -> w323
              tunnel: w320 -> [w326 w328]
              tunnel: w319 -> [w325 _]
              tunnel: w316 -> [w324 _]
              frame True {
                n127 = invoke class="VI" method="FP.Open"(reference=w325, error in=w326, "State"=w324) -> (error out=w327:errorcluster)  [unwired: 2 in, 4 out]
              }
              frame False {
              }
            }
          }
        }
        n128 = call <vilib>:"Add State(s) to Queue__JKI_lib_State_Machine.vi"("State(s) in (\"\")"=w263) -> ("States Out"=w262:string)  [unwired: 14 in]
      }
      frame "UI: Post Action" {
        n129 = Unbundle By Name(w339) -> ("Polish.Hold"=w337:bool, "Polish.2D Picture"=w335:refnum<vi>, "Polish.Slides"=w334:picture[], "Polish.Action"=w342:refnum<vi>, "Polish.Progress Bar"=w344:refnum<vi>)
        n130 = property on="Property Node" class="LstBox (strict)"(reference=w346) -> (reference out=w348:refnum<vi>, error out=w347:errorcluster, "Value"=w338:i32, "Item Symbols"=w356:i32[], "Item Names"=w345:string[])  [unwired: 1 in]
        n131 = call "Periodic Trigger (OpenG).vi"("Time (ms)"=u32 3000 ("time (ms)")) -> ("Triggered"=w332:bool)  [unwired: 12 in, 2 out]
        n132 = Not(x=w337) -> (.not. x?=w340:bool)
        n133 = And(x=w332, y=w340) -> (x .and. y?=w336:bool)
        n134 = case shown="True" w336 {
          tunnel: w335 -> [_ w366]
          tunnel: w334 -> [_ w362]
          frame False {
          }
          frame True {
            n135 = property class="Pict"(reference=w366) -> (reference out=w361:refnum<vi>, "Value"=w365:picture)  [unwired: 1 in, 1 out]
            n136 = Array Size(array=w362) -> (size(s)=w358:i32)
            n137 = Search 1D Array(1D array=w362, element=w365) -> (index of element=w364:i32)  [unwired: 1 in]
            n138 = Increment(x=w364) -> (x+1=w359:i32)
            n139 = Quotient & Remainder(x=w359, y=w358) -> (x-y*floor(x/y)=w363:i32)  [unwired: 1 out]
            n140 = Index Array(array=w362, index=w363) -> (element=w360:picture)
            n141 = property class="Pict"(reference=w361, "Value"=w360) -> ()  [unwired: 1 in, 2 out]
          }
        }
        n142 = Replace Array Subset(array=w356, new element=1 ("new element/subarray"), index=w338) -> (w354:i32[])
        n143 = Subtract(x=w338, y=5) -> (x-y=w351:i32)
        n144 = Increment(x=w338) -> (x+1=w343:i32)
        n145 = Increment(x=w338) -> (x+1=w329:i32)
        n146 = Increment(x=w338) -> (x+1=w353:i32)
        n147 = property class="Slide (strict)"(reference=w344, "Value"=w343) -> ()  [unwired: 1 in, 2 out]
        n148 = Max & Min(x=w351, y=0) -> (max(x,y)=w349:i32)  [unwired: 1 out]
        n149 = Index Array(array=w345, index=w329) -> (element=w341:string)
        n150 = property on="Property Node" class="LstBox (strict)"(reference=w348, error in=w347, "Top Row"=w349, "Item Symbols"=w354, "Value"=w353) -> ()  [unwired: 2 out]
        n151 = property class="Str"(reference=w342, "Value"=w341) -> ()  [unwired: 1 in, 2 out]
        n152 = call <vilib>:"Add State(s) to Queue__JKI_lib_State_Machine.vi"("State(s) in (\"\")"=w330) -> ("States Out"=w331:string)  [unwired: 14 in]
      }
      frame "---------- Macro ----------" {
        # "Do not put any code in this frame.\n(It is a separator no-op. You can make a copy of this frame to create a new Macro frame)"
        n153 = call <vilib>:"Add State(s) to Queue__JKI_lib_State_Machine.vi"("State(s) in (\"\")"=w370) -> ("States Out"=w369:string)  [unwired: 14 in]
      }
      frame "Macro: Initialize" {
        # "Initialization Macro\n(This is called once, when the VI starts)"
        n154 = call <vilib>:"Add State(s) to Queue__JKI_lib_State_Machine.vi"("State(s) in Front (\"\")"="Data: Initialize\nData: InitializePolish\nInitialize Core Data\nData: List all lvclasses\nData: List all _JKI State Machine Helper VIs\nData: List all _JKI State Machine Helper Folders\nData: List all CSM Templates\nUI: Initialize\nUI: Front Panel State >> Open\nUI: Bring Window to Topmost(Windows Only)\nInitialize: Append steps of fixing JKISM Editor in MultiListbox\n//Initialize: Append Simplify lvclass steps in Multilistbox\n//UI: Append Item to Multilistbox >> Refersh More Template palette\n//Initialize: Append Mass Compile Steps in MultiListbox\nInitialize: Append steps of et_csm_doc_case_as_default\n//github #330 https://github.com/NEVSTOP-LAB/Communicable-State-Machine/issues/330\n//Macro: Localize CSM\nMacro: Open VI for recompile\nInsert Task >> Refresh Popup Menus\nUI: Refresh Listbox\nMacro: Set Toolbar Entry Run when Opened\n\nFix for Linux: JKISM VI missing in Palette\n\n//---------------\nMacro: Start\n//---------------\nMacro: Exit", "State(s) in (\"\")"=w375) -> ("States Out"=w374:string)  [unwired: 13 in]
      }
      frame "Macro: Start" {
        n155 = Unbundle By Name(w380) -> ("Actions"=w379:string[])
        n156 = call "CSM - Compact Multiple States.vi"("Multiple States"=w379) -> ("States"=w376:string)  [unwired: 9 in]
        n157 = call <vilib>:"Add State(s) to Queue__JKI_lib_State_Machine.vi"("State(s) in Front (\"\")"=w376, "State(s) in (\"\")"=w377) -> ("States Out"=w378:string)  [unwired: 13 in]
      }
      frame "Macro: Open VI for recompile" {
        n158 = Build Array("_xnode" ("name or relative path"), "_csmHelper" ("name or relative path"), "_popupMenuPlugin" ("name or relative path"), "_tool" ("name or relative path")) -> (w388:string[])
        n159 = for {
          tunnel: w388 -> [w403] mode=indexing
          tunnel: [w397] -> w389 mode=concatenating
          n160 = call "CSM - user.lib Dir.vi"() -> ("csm_user.lib_dir"=w396:path)  [unwired: 2 in, 1 out]
          n161 = Build Path(base path=w396, name or relative path=w403) -> (appended path=w402:path)
          n162 = call <vilib>:"Recursive File List.vi"("pattern"="*.vi", "Continue Recursing on Error? (F)"=TRUE ("Treat LLBs as Folders?"), "Treat LLBs as Folders?"=FALSE, "Folder Path"=w402) -> ("All Files in Dir"=w399:path[])  [unwired: 3 in, 4 out]
          n163 = for {
            tunnel: w399 -> [w407] mode=indexing
            tunnel: [w408] -> w400 mode=indexing
            tunnel: w396 -> [w406]
            n164 = call <vilib>:"Compare Two Paths.vi"("Path 2"=w407, "Path 1"=w406) -> ("Relative Path from 1 to 2"=w405:path)  [unwired: 6 in, 3 out]
            n165 = Path To String(path=w405) -> (string=w404:string)
            n166 = call <vilib>:"Build State String with Arguments__JKI_lib_State_Machine.vi"("Arguments (\"\")"=w404, "State"="Open VIRef to Compile CSM Tools") -> ("State with Arguments"=w410:string)  [unwired: 4 in]
            n167 = call <vilib>:"Build State String with Arguments__JKI_lib_State_Machine.vi"("Arguments (\"\")"=w410, "State"="Insert Task") -> ("State with Arguments"=w408:string)  [unwired: 4 in]
          }
          n168 = Reverse 1D Array(array=w400) -> (reversed array=w397:string[])
        }
        n169 = call "CSM - Compact Multiple States.vi"("Multiple States"=w389) -> ("States"=w385:string)  [unwired: 9 in]
        n170 = call <vilib>:"Add State(s) to Queue__JKI_lib_State_Machine.vi"("State(s) in (\"\")"="UI: Bring Window to Topmost(Windows Only)\nInsert Task >> Open VIRef to Compile CSM Tools2  >> user.lib\\_NEVSTOP\\Communicable State Machine(CSM)\\CSM User Interface(UI) Module Template.vi\nInsert Task >> Open VIRef to Compile CSM Tools2 >> user.lib\\_NEVSTOP\\Communicable State Machine(CSM)\\CSM Module Template.vi\nInsert Task >> Open VIRef to Compile CSM Tools2 >> templates\\Communicable State Machine(CSM)\\CSM DQMH-Style Template.vi\nInsert Task >> Open VIRef to Compile CSM Tools2 >> templates\\Communicable State Machine(CSM)\\CSM Module Template - Tiny.vi\nInsert Task >> Open VIRef to Compile CSM Tools2 >> templates\\Communicable State Machine(CSM)\\CSM User Interface(UI) Module Template - Tiny.vi" ("State(s) in Front (\"\")"), "State(s) at Back (\"\")"=w385) -> ("States Out"=w386:string)  [unwired: 13 in]
        n171 = call <vilib>:"Add State(s) to Queue__JKI_lib_State_Machine.vi"("State(s) in Front (\"\")"=w386, "State(s) in (\"\")"=w391) -> ("States Out"=w392:string)  [unwired: 13 in]
      }
      frame "Macro: Run CSM to Recompile" {
        n172 = call <vilib>:"Add State(s) to Queue__JKI_lib_State_Machine.vi"("State(s) in (\"\")"="Insert Task >> Run Template to Compile CSM API >> user.lib\\_NEVSTOP\\Communicable State Machine(CSM)\\CSM User Interface(UI) Module Template.vi\nInsert Task >> Run Template to Compile CSM API >> user.lib\\_NEVSTOP\\Communicable State Machine(CSM)\\CSM Module Template.vi\nInsert Task >> Run Template to Compile CSM API >> templates\\Communicable State Machine(CSM)\\CSM DQMH-Style Template.vi\nInsert Task >> Run Template to Compile CSM API >> templates\\Communicable State Machine(CSM)\\CSM Module Template - Tiny.vi\nInsert Task >> Run Template to Compile CSM API >> templates\\Communicable State Machine(CSM)\\CSM User Interface(UI) Module Template - Tiny.vi" ("State(s) in Front (\"\")")) -> ("States Out"=w412:string)  [unwired: 14 in]
        n173 = call <vilib>:"Add State(s) to Queue__JKI_lib_State_Machine.vi"("State(s) in Front (\"\")"=w412, "State(s) in (\"\")"=w414) -> ("States Out"=w415:string)  [unwired: 13 in]
      }
      frame "Macro: Localize CSM" {
        n174 = call <vilib>:"Add State(s) to Queue__JKI_lib_State_Machine.vi"("State(s) in (\"\")"="//Insert Task >> Check System Language\n//Insert Task >> Load Localization Files\n//Initialize: Localize All VIs\n//UI: Bring Window to Topmost(Windows Only)" ("State(s) in Front (\"\")")) -> ("States Out"=w418:string)  [unwired: 14 in]
        n175 = call <vilib>:"Add State(s) to Queue__JKI_lib_State_Machine.vi"("State(s) in Front (\"\")"=w418, "State(s) in (\"\")"=w420) -> ("States Out"=w421:string)  [unwired: 13 in]
      }
      frame "Macro: Set Toolbar Entry Run when Opened" {
        n176 = call "_script_enable_run_when_opened.vi"() -> ("error out"=w424:errorcluster)  [unwired: 11 in]
        n177 = call <vilib>:"Clear Errors.vi"("error in (no error)"=w424) -> ()  [unwired: 5 in, 2 out]
      }
      frame "Macro: Exit" {
        # "Exit Macro\n(This is called once, when the VI exits)"
        n178 = Unbundle By Name(w434) -> ("Core.Close Panel on Exit?"=w433:bool)
        n179 = Select(t="UI: Front Panel State >> Close", s=w433, f="") -> (s? t:f=w430:string)
        n180 = call <vilib>:"Add State(s) to Queue__JKI_lib_State_Machine.vi"("State(s) in (\"\")"=w430, "State(s) at Back (\"\")"="Data: Cleanup\nExit") -> ("States Out"=w428:string)  [unwired: 13 in]
        n181 = call <vilib>:"Add State(s) to Queue__JKI_lib_State_Machine.vi"("State(s) in Front (\"\")"=w428, "State(s) in (\"\")"=w437) -> ("States Out"=w436:string)  [unwired: 13 in]
      }
      frame "---------------- Initialize ----------------" {
      }
      frame "Initialize: Append Recompile Steps in MultiListbox" {
        n182 = Unbundle By Name(w448) -> ("Actions"=w442:string[], "_JKI State Machine Helper VIs"=w447:path[])
        n183 = VI Library() -> (path=w445:path)
        n184 = Strip Path(path=w445) -> (stripped path=w444:path)  [unwired: 1 out]
        n185 = for {
          tunnel: w447 -> [w452] mode=indexing
          tunnel: [w453] -> w449 mode=indexing
          tunnel: w444 -> [w451]
          n186 = call <vilib>:"Compare Two Paths.vi"("Path 2"=w452, "Path 1"=w451) -> ("Relative Path from 1 to 2"=w454:path)  [unwired: 6 in, 3 out]
          n187 = Format Into String(format string="Recompile >> %s", w454) -> (resulting string=w453:string)  [unwired: 2 in, 1 out]
        }
        n188 = Build Array (concatenate)(w442, w449) -> (w441:string[])
        n189 = Bundle By Name(cluster=w448, "Actions"=w441) -> (w443:T3)
      }
      frame "Initialize: Append steps of fixing JKISM Editor in MultiListbox" {
        n190 = Unbundle By Name(w460) -> ("Actions"=w458:string[])
        n191 = Build Array (concatenate)(w458, string[] ["Fix JKISM Editor: fix_vi broken in Tree__JKI_State_Machine_Helper.vi", "Fix JKISM Editor: fix_Parse State Queue in Find Parse State Queue vi name.vi", "Fix JKISM Editor: fix_Parse State Queue in Find Parse State Queue vi name2.vi", "Fix JKISM Editor: Fix fix_exclude event case ref check.vi", "Fix JKISM Editor: fix_Find Event Stucture Ref vi.vi", "Fix JKISM Editor: fix_list event frames.vi"] ("element")) -> (w457:string[])
        n192 = Bundle By Name(cluster=w460, "Actions"=w457) -> (w459:T3)
      }
      frame "Initialize: Append Simplify lvclass steps in Multilistbox" {
        n193 = Unbundle By Name(w469) -> ("Actions"=w463:string[], "CSM lvclass"=w468:path[])
        n194 = call "CSM - user.lib Dir.vi"() -> ("<LabVIEW>"=w466:path)  [unwired: 2 in, 1 out]
        n195 = for {
          tunnel: w468 -> [w472] mode=indexing
          tunnel: [w476] -> w470 mode=indexing
          tunnel: w466 -> [w473]
          n196 = call <vilib>:"Compare Two Paths.vi"("Path 2"=w472, "Path 1"=w473) -> ("Relative Path from 1 to 2"=w474:path)  [unwired: 6 in, 3 out]
          n197 = Format Into String(format string="Clear lvclass mutation history >> %s", w474) -> (resulting string=w476:string)  [unwired: 2 in, 1 out]
        }
        n198 = Build Array (concatenate)(w463, w470) -> (w464:string[])
        n199 = Bundle By Name(cluster=w469, "Actions"=w464) -> (w465:T3)
      }
      frame "Initialize: Append Mass Compile Steps in MultiListbox" {
        n200 = Unbundle By Name(w485) -> ("Actions"=w479:string[], "_JKI State Machine Helper Folders"=w484:path[])
        n201 = VI Library() -> (path=w482:path)
        n202 = Strip Path(path=w482) -> (stripped path=w481:path)  [unwired: 1 out]
        n203 = for {
          tunnel: w484 -> [w487] mode=indexing
          tunnel: [w489] -> w477 mode=indexing
          tunnel: w481 -> [w488]
          n204 = call <vilib>:"Compare Two Paths.vi"("Path 2"=w487, "Path 1"=w488) -> ("Relative Path from 1 to 2"=w490:path)  [unwired: 6 in, 3 out]
          n205 = Format Into String(format string="Mass Compile >> %s", w490) -> (resulting string=w489:string)  [unwired: 2 in, 1 out]
        }
        n206 = Build Array (concatenate)(w479, w477) -> (w478:string[])
        n207 = Bundle By Name(cluster=w485, "Actions"=w478) -> (w480:T3)
      }
      frame "Initialize: Append steps of et_csm_doc_case_as_default" {
        n208 = Unbundle By Name(w498) -> ("Actions"=w492:string[], "CSM Templates"=w497:path[])
        n209 = call "CSM - user.lib Dir.vi"() -> ("<LabVIEW>"=w495:path)  [unwired: 2 in, 1 out]
        n210 = for {
          tunnel: w497 -> [w502] mode=indexing
          tunnel: [w503] -> w499 mode=indexing
          tunnel: w495 -> [w501]
          n211 = call <vilib>:"Compare Two Paths.vi"("Path 2"=w502, "Path 1"=w501) -> ("Relative Path from 1 to 2"=w504:path)  [unwired: 6 in, 3 out]
          n212 = Format Into String(format string="Set First CSM Case >> %s", w504) -> (resulting string=w503:string)  [unwired: 2 in, 1 out]
        }
        n213 = Build Array (concatenate)(w492, w499) -> (w493:string[])
        n214 = Bundle By Name(cluster=w498, "Actions"=w493) -> (w494:T3)
      }
      frame "Initialize: Append Item to Multilistbox", "Insert Task" {
        n215 = Unbundle By Name(w510) -> ("Actions"=w508:string[])
        n216 = Build Array(w512) -> (w511:string[])
        n217 = Build Array (concatenate)(w508, w511) -> (w507:string[])
        n218 = Bundle By Name(cluster=w510, "Actions"=w507) -> (w509:T3)
      }
      frame "Initialize: Localize All VIs" {
        n219 = call "CSM - user.lib Dir.vi"() -> ("<LabVIEW>"=w517:path)  [unwired: 2 in, 1 out]
        n220 = Unbundle By Name(w525) -> ("Actions"=w521:string[])
        n221 = Path to Array of Strings(0:w517) -> (2:w519:string[])  [unwired: 1 out]
        n222 = call "_list_CSM documented VIs.vi"() -> ("Array"=w520:path[])  [unwired: 11 in]
        n223 = Array Size(array=w519) -> (size(s)=w518:i32)
        n224 = for {
          tunnel: w520 -> [w533] mode=indexing
          tunnel: w518 -> [w531]
          tunnel: [w530] -> w516 mode=indexing
          n225 = Path to Array of Strings(0:w533) -> (2:w532:string[])  [unwired: 1 out]
          n226 = Array Subset(array=w532, index=w531) -> (w529:string[])  [unwired: 1 in]
          n227 = Array of Strings to Path(0:w529, 1:TRUE ("relative")) -> (2:w530:path)
        }
        n228 = Path To String(path=w516) -> (string=w514:string[])
        n229 = for {
          tunnel: [w536] -> w526 mode=indexing
          tunnel: "Localize VI Description >> %s" ("format string") -> [w535]
          tunnel: w514 -> [w534] mode=indexing
          n230 = Format Into String(format string=w535, w534) -> (resulting string=w536:string)  [unwired: 2 in, 1 out]
        }
        n231 = Build Array (concatenate)(w521, w526) -> (w522:string[])
        n232 = Bundle By Name(cluster=w525, "Actions"=w522) -> (w523:T3)
      }
      frame "---------- Action ----------" {
        # "Template Separator\n(You can make a copy of, or modify, this frame)"
        n233 = call <vilib>:"Add State(s) to Queue__JKI_lib_State_Machine.vi"("State(s) in (\"\")"=w540) -> ("States Out"=w539:string)  [unwired: 14 in]
      }
      frame "Recompile" {
        n234 = call "String to Path.vi"("String"=w545) -> ("Path"=w544:path)
        n235 = Open VI Reference(vi path=w544) -> (vi reference=w551:refnum<vi>, error out=w552:errorcluster)  [unwired: 5 in]
        n236 = invoke class="VI" method="Compile"(reference=w551, error in=w552, "Entire Hierarchy"=FALSE ("Compile Entire Hierarchy (F)"), "Force Compile"=TRUE ("Force Compile (T)")) -> (reference out=w550:refnum<vi>, error out=w549:errorcluster)  [unwired: 1 in, 3 out]
        n237 = invoke class="VI" method="Save.Instrument"(reference=w550, error in=w549) -> (reference out=w547:refnum<vi>, error out=w548:errorcluster)  [unwired: 4 in, 4 out]
        n238 = Close Reference(reference=w547, error in (no error)=w548) -> (error out=w546:errorcluster)
        n239 = call <vilib>:"Clear Errors.vi"("error in (no error)"=w546) -> ()  [unwired: 5 in, 2 out]
        n240 = call <vilib>:"Add State(s) to Queue__JKI_lib_State_Machine.vi"("State(s) in Front (\"\")"="UI: Post Action" ("State(s) in Front (\"\")"), "State(s) in (\"\")"=w542) -> ("States Out"=w543:string)  [unwired: 13 in]
      }
      frame "Set First CSM Case" {
        n241 = call "String to Path.vi"("String"=w558) -> ("Path"=w557:path)
        n242 = call "CSM - user.lib Dir.vi"() -> ("<LabVIEW>"=w560:path)  [unwired: 2 in, 1 out]
        n243 = Build Path(base path=w560, name or relative path=w557) -> (appended path=w559:path)
        n244 = call "_script_set_csm_doc_case_as_default.vi"("Vi Path"=w559) -> ("error out"=w564:errorcluster)  [unwired: 10 in]
        n245 = call <vilib>:"Clear Errors.vi"("error in (no error)"=w564) -> ()  [unwired: 5 in, 2 out]
        n246 = call <vilib>:"Add State(s) to Queue__JKI_lib_State_Machine.vi"("State(s) in Front (\"\")"="UI: Post Action" ("State(s) in Front (\"\")"), "State(s) in (\"\")"=w562) -> ("States Out"=w563:string)  [unwired: 13 in]
      }
      frame "Clear lvclass mutation history" {
        n247 = call "String to Path.vi"("String"=w568) -> ("Path"=w567:path)
        n248 = call "CSM - user.lib Dir.vi"() -> ("<LabVIEW>"=w570:path)  [unwired: 2 in, 1 out]
        n249 = Build Path(base path=w570, name or relative path=w567) -> (appended path=w569:path)
        n250 = call "clear the mutation history for the classes.vi"("Path"=w569) -> ()  [unwired: 11 in]
        n251 = call <vilib>:"Add State(s) to Queue__JKI_lib_State_Machine.vi"("State(s) in Front (\"\")"="UI: Post Action" ("State(s) in Front (\"\")"), "State(s) in (\"\")"=w572) -> ("States Out"=w573:string)  [unwired: 13 in]
      }
      frame "Fix JKISM Editor: fix_Parse State Queue in Find Parse State Queue vi name.vi" {
        n252 = call "_script_fix_Parse State Queue in Find Parse State Queue vi name.vi"() -> ()  [unwired: 12 in]
        n253 = call <vilib>:"Add State(s) to Queue__JKI_lib_State_Machine.vi"("State(s) in Front (\"\")"="UI: Post Action" ("State(s) in Front (\"\")"), "State(s) in (\"\")"=w577) -> ("States Out"=w578:string)  [unwired: 13 in]
      }
      frame "Fix JKISM Editor: fix_Parse State Queue in Find Parse State Queue vi name2.vi" {
        n254 = call "_script_fix_Parse State Queue in Find Parse State Queue vi name2.vi"() -> ()  [unwired: 12 in]
        n255 = call <vilib>:"Add State(s) to Queue__JKI_lib_State_Machine.vi"("State(s) in Front (\"\")"="UI: Post Action" ("State(s) in Front (\"\")"), "State(s) in (\"\")"=w582) -> ("States Out"=w583:string)  [unwired: 13 in]
      }
      frame "Fix JKISM Editor: fix_vi broken in Tree__JKI_State_Machine_Helper.vi" {
        n256 = call "_script_fix_vi broken in Tree__JKI_State_Machine_Helper.vi"() -> ()  [unwired: 12 in]
        n257 = call <vilib>:"Add State(s) to Queue__JKI_lib_State_Machine.vi"("State(s) in Front (\"\")"="UI: Post Action" ("State(s) in Front (\"\")"), "State(s) in (\"\")"=w587) -> ("States Out"=w588:string)  [unwired: 13 in]
      }
      frame "Fix JKISM Editor: Fix fix_exclude event case ref check.vi" {
        n258 = call "_script_fix_exclude event case ref check.vi"() -> ()  [unwired: 12 in]
        n259 = call <vilib>:"Add State(s) to Queue__JKI_lib_State_Machine.vi"("State(s) in Front (\"\")"="UI: Post Action" ("State(s) in Front (\"\")"), "State(s) in (\"\")"=w592) -> ("States Out"=w593:string)  [unwired: 13 in]
      }
      frame "Fix JKISM Editor: fix_Find Event Stucture Ref vi.vi" {
        n260 = call "_script_fix_Find Event Stucture Ref vi.vi"() -> ()  [unwired: 12 in]
        n261 = call <vilib>:"Add State(s) to Queue__JKI_lib_State_Machine.vi"("State(s) in Front (\"\")"="UI: Post Action" ("State(s) in Front (\"\")"), "State(s) in (\"\")"=w597) -> ("States Out"=w598:string)  [unwired: 13 in]
      }
      frame "Fix JKISM Editor: fix_list event frames.vi" {
        n262 = call "_script_fix_list event frames.vi"() -> ()  [unwired: 12 in]
        n263 = call <vilib>:"Add State(s) to Queue__JKI_lib_State_Machine.vi"("State(s) in Front (\"\")"="UI: Post Action" ("State(s) in Front (\"\")"), "State(s) in (\"\")"=w602) -> ("States Out"=w603:string)  [unwired: 13 in]
      }
      frame "Fix for Linux: JKISM VI missing in Palette" {
        n264 = call "_fix_linux_palette_path_issue.vi"() -> ()  [unwired: 12 in]
        n265 = call <vilib>:"Add State(s) to Queue__JKI_lib_State_Machine.vi"("State(s) in Front (\"\")"="UI: Post Action" ("State(s) in Front (\"\")"), "State(s) in (\"\")"=w607) -> ("States Out"=w608:string)  [unwired: 13 in]
      }
      frame "Mass Compile" {
        n266 = call "String to Path.vi"("String"=w612) -> ("Path"=w611:path)
        n267 = call "CSM - user.lib Dir.vi"() -> ("<LabVIEW>"=w614:path)  [unwired: 2 in, 1 out]
        n268 = Build Path(base path=w614, name or relative path=w611) -> (appended path=w613:path)
        n269 = invoke class="App" method="Mass Compile"("Directory to Compile"=w613) -> (error out=w620:errorcluster)  [unwired: 8 in, 8 out]
        n270 = call <vilib>:"Clear Errors.vi"("error in (no error)"=w620) -> ()  [unwired: 5 in, 2 out]
        n271 = Wait (ms)(milliseconds to wait=u32 1000) -> ()  [unwired: 1 out]
        n272 = call <vilib>:"Add State(s) to Queue__JKI_lib_State_Machine.vi"("State(s) in Front (\"\")"="UI: Post Action" ("State(s) in Front (\"\")"), "State(s) in (\"\")"=w616) -> ("States Out"=w617:string)  [unwired: 13 in]
      }
      frame "Run Template to Compile CSM API" {
        n273 = call "CSM - user.lib Dir.vi"() -> ("<LabVIEW>"=w623:path)  [unwired: 2 in, 1 out]
        n274 = call "String to Path.vi"("String"=w624) -> ("Path"=w622:path)
        n275 = Build Path(base path=w623, name or relative path=w622) -> (appended path=w627:path)
        n276 = call <vilib>:"Check if File or Folder Exists.vi"("path"=w627) -> ("file or folder exists?"=w625:bool, "dup path"=w626:path)  [unwired: 8 in, 1 out]
        n277 = case shown="True" w625 {
          tunnel: w626 -> [w633 w636]
          frame False {
            n278 = Path To String(path=w633) -> (string=w634:string)
            n279 = Two Button Dialog(message=w634, 2:"Ack" ("T button name (\"OK\")")) -> ()  [unwired: 1 in, 1 out]
          }
          frame True {
            n280 = call "uuid.vi"() -> ("UUID"=w639:string)  [unwired: 11 in]
            n281 = Open VI Reference(type specifier VI Refnum (for type only)=refnum<vi> refnum, vi path=w636, options=128) -> (vi reference=w643:refnum<vi>, error out=w644:errorcluster)  [unwired: 3 in]
            n282 = call-by-ref "Start Asynchronous Call"(reference=w643, error in=w644, "Name(\"\" to use uuid)"=w639) -> (reference out=w646:refnum<vi>, error out=w645:errorcluster)  [unwired: 11 in]
            n283 = Close Reference(reference=w646, error in (no error)=w645) -> (error out=w641:errorcluster)
            n284 = flat-sequence {
              tunnel: w641 -> [w648]
              tunnel: [w648] -> w640
              frame #0 {
                n285 = Wait (ms)(milliseconds to wait=u32 500) -> ()  [unwired: 1 out]
              }
            }
            n286 = call "CSM - Send Message and Wait for Reply.vi"("Error In (No Error)"=w640, "Target Module"=w639, "State"="Macro: Exit") -> ("error out"=w637:errorcluster)  [unwired: 6 in, 2 out]
            n287 = call <vilib>:"Clear Errors.vi"("error in (no error)"=w637) -> ()  [unwired: 5 in, 2 out]
          }
        }
        n288 = call <vilib>:"Add State(s) to Queue__JKI_lib_State_Machine.vi"("State(s) in Front (\"\")"="UI: Post Action" ("State(s) in Front (\"\")"), "State(s) in (\"\")"=w629) -> ("States Out"=w630:string)  [unwired: 13 in]
      }
      frame "Open VIRef to Compile CSM Tools" {
        n289 = call "CSM - user.lib Dir.vi"() -> ("csm_user.lib_dir"=w655:path)  [unwired: 2 in, 1 out]
        n290 = call "String to Path.vi"("String"=w651) -> ("Path"=w650:path)
        n291 = Build Path(base path=w655, name or relative path=w650) -> (appended path=w656:path)
        n292 = call <vilib>:"Check if File or Folder Exists.vi"("path"=w656) -> ("error out"=w654:errorcluster, "file or folder exists?"=w653:bool, "dup path"=w652:path)  [unwired: 8 in]
        n293 = case shown="True" w653 {
          tunnel: w654 -> [_ w667]
          tunnel: w652 -> [w663 w666]
          frame False {
            n294 = Path To String(path=w663) -> (string=w662:string)
            n295 = Two Button Dialog(message=w662, 2:"Ack" ("T button name (\"OK\")")) -> ()  [unwired: 1 in, 1 out]
          }
          frame True {
            n296 = call "Open VIRef to Compile.vi"("error in (no error)"=w667, "milliseconds to wait"=u32 20, "dup path"=w666) -> ("error out"=w668:errorcluster)  [unwired: 8 in]
            n297 = call <vilib>:"Clear Errors.vi"("error in (no error)"=w668) -> ()  [unwired: 5 in, 2 out]
          }
        }
        n298 = call <vilib>:"Add State(s) to Queue__JKI_lib_State_Machine.vi"("State(s) in Front (\"\")"="UI: Post Action" ("State(s) in Front (\"\")"), "State(s) in (\"\")"=w658) -> ("States Out"=w659:string)  [unwired: 13 in]
      }
      frame "Open VIRef to Compile CSM Tools2" {
        n299 = call "String to Path.vi"("String"=w671) -> ("Path"=w669:path)
        n300 = call "CSM - user.lib Dir.vi"() -> ("<LabVIEW>"=w670:path)  [unwired: 2 in, 1 out]
        n301 = Build Path(base path=w670, name or relative path=w669) -> (appended path=w675:path)
        n302 = call <vilib>:"Check if File or Folder Exists.vi"("path"=w675) -> ("error out"=w674:errorcluster, "file or folder exists?"=w673:bool, "dup path"=w672:path)  [unwired: 8 in]
        n303 = case shown="True" w673 {
          tunnel: w674 -> [_ w685]
          tunnel: w672 -> [w682 w686]
          frame False {
            n304 = Path To String(path=w682) -> (string=w681:string)
            n305 = Two Button Dialog(message=w681, 2:"Ack" ("T button name (\"OK\")")) -> ()  [unwired: 1 in, 1 out]
          }
          frame True {
            n306 = call "Open VIRef to Compile.vi"("error in (no error)"=w685, "milliseconds to wait"=u32 20, "dup path"=w686) -> ("error out"=w684:errorcluster)  [unwired: 8 in]
            n307 = call <vilib>:"Clear Errors.vi"("error in (no error)"=w684) -> ()  [unwired: 5 in, 2 out]
          }
        }
        n308 = call <vilib>:"Add State(s) to Queue__JKI_lib_State_Machine.vi"("State(s) in Front (\"\")"="UI: Post Action" ("State(s) in Front (\"\")"), "State(s) in (\"\")"=w677) -> ("States Out"=w678:string)  [unwired: 13 in]
      }
      frame "Refresh Popup Menus" {
        n309 = VI Library() -> (path=w696:path)
        n310 = Strip Path(path=w696) -> (stripped path=w695:path)  [unwired: 1 out]
        n311 = Build Path(base path=w695, name or relative path=path "resource/plugins/PopupMenus/support/Refresh Menus.vi") -> (appended path=w694:path)
        n312 = call <vilib>:"Check if File or Folder Exists.vi"("path"=w694) -> ("file or folder exists?"=w692:bool, "dup path"=w693:path)  [unwired: 8 in, 1 out]
        n313 = case shown="True" w692 {
          tunnel: w693 -> [_ w705]
          frame False {
          }
          frame True {
            n314 = Open VI Reference(vi path=w705) -> (vi reference=w704:refnum<vi>, error out=w703:errorcluster)  [unwired: 5 in]
            n315 = invoke class="VI" method="Run VI"(reference=w704, error in=w703, "Wait until done"=TRUE ("Wait Until Done"), "Auto Dispose Ref"=FALSE ("Auto Dispose Reference")) -> (reference out=w699:refnum<vi>, error out=w700:errorcluster)  [unwired: 1 in, 3 out]
            n316 = Close Reference(reference=w699, error in (no error)=w700) -> ()  [unwired: 1 out]
          }
        }
        n317 = call <vilib>:"Add State(s) to Queue__JKI_lib_State_Machine.vi"("State(s) in Front (\"\")"="UI: Post Action" ("State(s) in Front (\"\")"), "State(s) in (\"\")"=w690) -> ("States Out"=w691:string)  [unwired: 13 in]
      }
      frame "Check System Language" {
        n318 = call "_csm_System_Language.vi"() -> ("LangID"=w709:string)  [unwired: 11 in]
        n319 = Bundle By Name(cluster=w711, "LangID"=w709) -> (w710:T3)
        n320 = call <vilib>:"Add State(s) to Queue__JKI_lib_State_Machine.vi"("State(s) in Front (\"\")"="UI: Post Action" ("State(s) in Front (\"\")"), "State(s) in (\"\")"=w707) -> ("States Out"=w708:string)  [unwired: 13 in]
      }
      frame "Load Localization Files" {
        w713 = variant ("DescMap")
        n321 = Unbundle By Name(w718) -> ()  [unwired: 1 out]
        n322 = Bundle By Name(cluster=w718, "DescMap"=w713, "NoteMap"=w713) -> (w717:T3)
        n323 = call <vilib>:"Add State(s) to Queue__JKI_lib_State_Machine.vi"("State(s) in Front (\"\")"="UI: Post Action" ("State(s) in Front (\"\")"), "State(s) in (\"\")"=w715) -> ("States Out"=w716:string)  [unwired: 13 in]
      }
      frame "Localize VI Description" {
        n324 = Unbundle By Name(w726) -> ("LangID"=w727:string, "DescMap"=w729:variant, "NoteMap"=w730:variant)
        n325 = call "CSM - user.lib Dir.vi"() -> ("<LabVIEW>"=w731:path)  [unwired: 2 in, 1 out]
        n326 = call "String to Path.vi"("String"=w721) -> ("Path"=w720:path)
        n327 = Build Path(base path=w731, name or relative path=w720) -> (appended path=w728:path)
        n328 = Strip Path(path=w728) -> (name=w736:string)  [unwired: 1 out]
        n329 = Get Variant Attribute(Variant=w729, name=w736, default value (empty Variant)="" ("String")) -> (found=w735:bool, value=w732:string, error out=w734:errorcluster)  [unwired: 1 in, 1 out]
        n330 = case shown="True" w735 {
          tunnel: w734 -> [w737 w740]
          tunnel: [w737 w741] -> w725
          tunnel: w732 -> [_ w738]
          tunnel: w730 -> [_ _]
          tunnel: w728 -> [_ w739]
          tunnel: w727 -> [_ _]
          frame False {
          }
          frame True {
            n331 = call "Populate Single VI Help.vi"("error in (no error)"=w740, "VI Description"=w738, "Path"=w739) -> ("error out"=w741:errorcluster)  [unwired: 8 in]
          }
        }
        n332 = call <vilib>:"Add State(s) to Queue__JKI_lib_State_Machine.vi"("State(s) in Front (\"\")"="UI: Post Action" ("State(s) in Front (\"\")"), "State(s) in (\"\")"=w723) -> ("States Out"=w724:string)  [unwired: 13 in]
      }
    }
  }
  n333 = call <vilib>:"Clear Errors.vi"("error in (no error)"=w1) -> ()  [unwired: 5 in, 2 out]
